vi "Tester.vi"(8 "error in (no error)":errorcluster, 11 "Selector in":refnum<class "Selector.lvclass">) -> (0 "error out":errorcluster, 3 "Selector out":refnum<class "Selector.lvclass">)   [LabVIEW 2019, in "Selector.lvclass"]
uses:
  Selector.lvclass
  Parse/ParseVectorFile/Typedefs/PrivateEvents--ParseVectorFile.NewFile.ctl
  <userlib>/Levylab/Relay Box/Typedefs/Resistor--enum.ctl
  Settings/ObjectSettings/ObjectSettings.lvclass/ObjectSettings.ctl
  Selector.lvclass/Selector.ctl
  <vilib>/Utility/miscctls.llb/LVPositionTypeDef.ctl
  Parse/ParseVectorFile/ParseVectorFile.lvclass
  C:/Program Files/National Instruments/LabVIEW 2019/vi.lib/JKI/JKI SMO/SMO/SMO.lvclass
  Settings/Setting Database/Setting Database.lvclass
  Subpanel/Manager/Subpanel.Edit.lvclass
  C:/Users/Albro/Documents/GitHub/AFM-Lithography/lvsrc/Classes/Subpanel/Subpanel.lvclass
  Tool/Tool Data/Tool Data/Tool Data.lvclass
  Render/BigMAQ/BigMAQ.lvclass
  Parse/ParsePaths/Path.lvclass
  Parse/Rectangle/Rectangle.lvclass
  Parse/Image/SVGImage.lvclass
  Parse/Dot/Dot.lvclass
  Settings/Setting Database/Typedefs/PublicEvents--Setting Database.RectanglesUpdated.ctl
  Settings/Rectangle Settings/Rectangle Settings.lvclass
  C:/Users/Albro/Documents/GitHub/AFM-Lithography/lvsrc/Classes/Settings/ObjectSettings/ObjectSettings.lvclass
  Settings/Setting Database/Typedefs/PublicEvents--Setting Database.PathsUpdated.ctl
  Settings/Path Settings/Path Settings.lvclass
  Settings/Setting Database/Typedefs/PublicEvents--Setting Database.FunnelsUpdated.ctl
  Settings/Funnel Settings/Funnel Settings.lvclass
  Settings/Setting Database/Typedefs/PublicEvents--Setting Database.DotsUpdated.ctl
  Settings/Dot Settings/Dot Settings.lvclass
  Tool/Tool Data/Tool Data/Typedefs/PrivateEvents--Tool Data.Update Objects.ctl
  Settings/Setting Database/Typedefs/PrivateEvents--Setting Database.Refresh.ctl
  Settings/Setting Database/Typedefs/PrivateEvents--Setting Database.Add To Group.ctl
  Settings/Setting Database/Typedefs/PrivateEvents--Setting Database.Create New Group.ctl
  Tool/Tool Path/Tool Path.lvclass
  Tool/Tool Funnel/Tool Funnel.lvclass
  Tool/Tool Rectangle/Tool Rectangle.lvclass
  Tool/Tool Dot/Tool Dots.lvclass
  <vilib>/JKI/JKI SMO/SMO/SMO.lvclass
  Settings/ObjectSettings/ObjectSettings.lvclass
  Subpanel/Subpanel.lvclass
  <userlib>/Levylab/Relay Box/Relay-Box.lvclass
  Identity/Identifier.lvclass
panel:
  in  "Collapse":bool
  out "Render":T1(plugin-control)
  in  "IBW":T2=path "C:/Users/Albro/Documents/GitHub/AFM-Lithography/test files/SA01234A0000.ibw"
  out "Lithography Data":T4(array[cluster])
  out "XY Graph":cluster{"X":dbl, "Y":dbl}[](graph)
  out "Array 2":i32[](array[numeric])
  out "Array":string[](array[string])
  out "Dots":string[](array[string])
  out "Funnels":string[](array[string])
  out "Paths":string[](array[string])
  out "Rectangles":string[](array[string])
  in  "NewFile":T2=path "C:/Users/Albro/Documents/GitHub/AFM-Lithography/test files/test.svg"
  out "Unchanged?":bool
  out "Events":string[](array[string])
  in  "Multicolumn Listbox":i32(listbox)
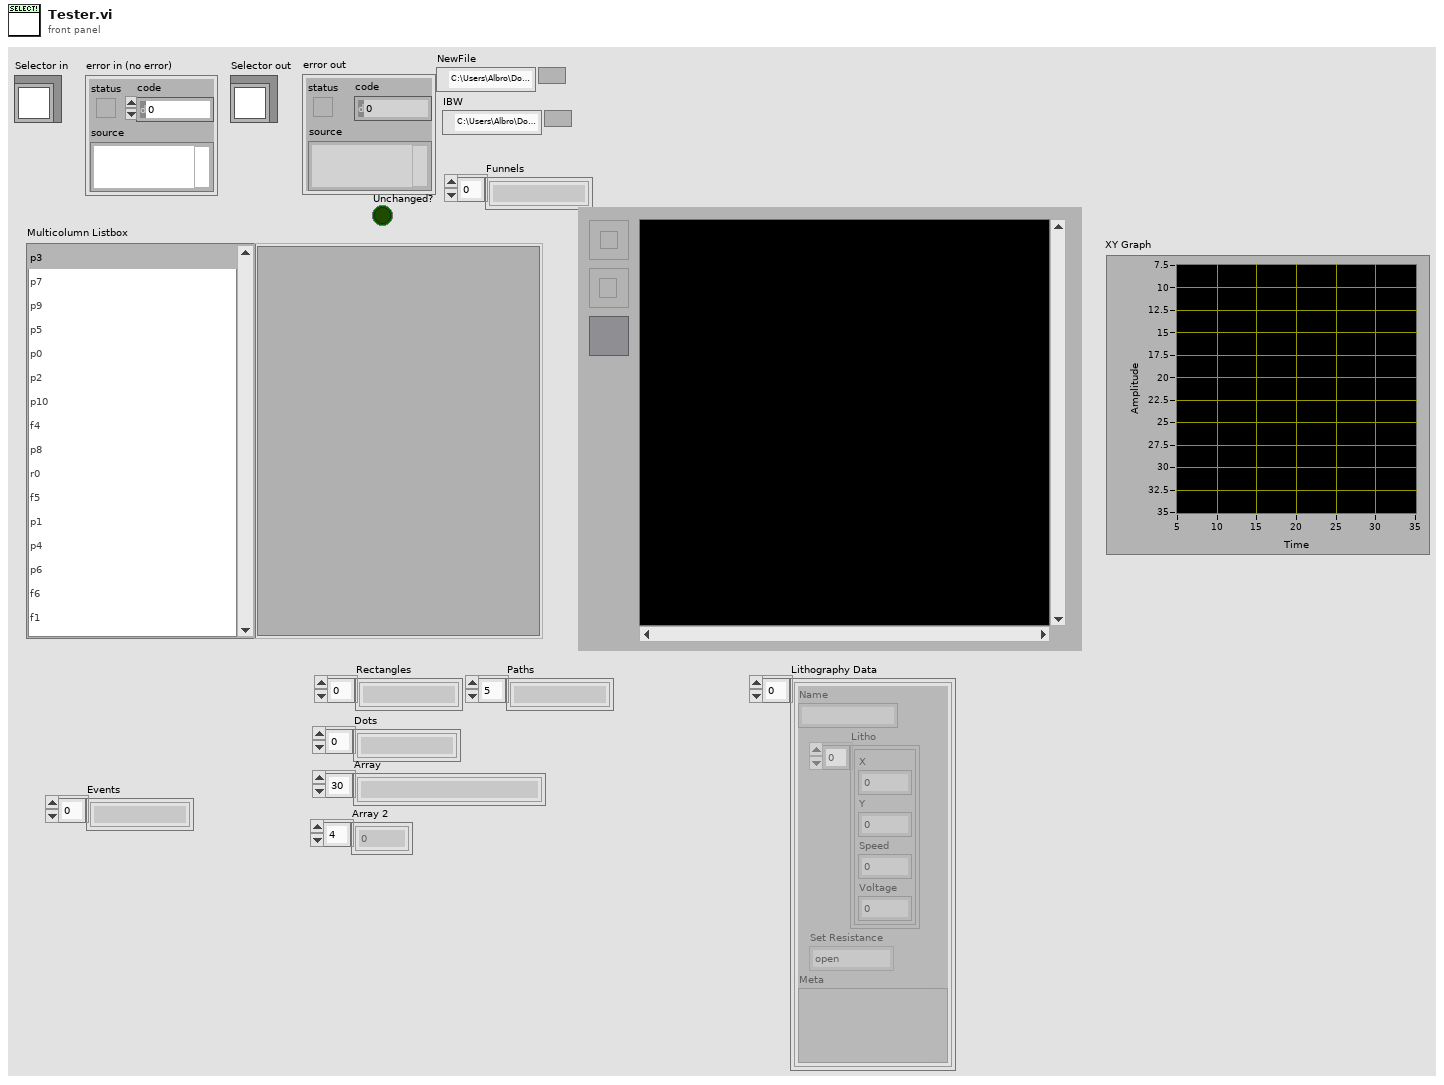
[diagram p1: front panel]
types:
  T1 = typedef "IMAQ Image.ctl" = refnum<image>
  T2 = typedef "ParseVectorFile.lvclass/PrivateEvents--ParseVectorFile.NewFile.ctl" = path
  T3 = typedef "Relay-Box.lvclass/Resistor--enum.ctl" = enum16{"open", "discharge tip", "0 ohms", "100k ohm", "10M ohm", "1G ohm"}
  T4 = cluster{"Name":string, "Litho":cluster{"X":dbl, "Y":dbl, "Speed":dbl, "Voltage":dbl}[], "Set Resistance":T3, "Meta":variant}[]
  T5 = typedef "LVPositionTypeDef.ctl" = cluster{"Left":i32, "Top":i32}
  T6 = cluster{"Point":T5, "Button":u16, "PlatMods":cluster{"Shift":bool, "Ctrl":bool, "Alt":bool, "Cmd":bool, "Opt":bool}}
  T7 = enum32{"Invalid", "Standard", "Closed", "Hidden", "Minimized", "Maximized"}
  T8 = enum32{"invalid app kind", "Development System", "Run Time System", "Student Edition", "Embedded LabVIEW", "Evaluation", "Custom"}
  T9 = cluster{"Name":string, "Group":string, "Enabled":bool}
  T10 = typedef "Tool Data.lvclass/PrivateEvents--Tool Data.Update Objects.ctl" = cluster{"Settings":cluster{"Paths":T11, "Rectangles":T12, "Funnels":T13, "Dots":T14}, "Data":cluster{"Paths":refnum<class "Path.lvclass">[], "Rectangles":refnum<class "Rectangle.lvclass">[], "SVGImage":refnum<class "SVGImage.lvclass">, "Dots":refnum<class "Dot.lvclass">[], "Funnels":refnum<class "Path.lvclass">[]}}
  T11 = typedef "Setting Database.lvclass/PublicEvents--Setting Database.PathsUpdated.ctl" = refnum<class "Path Settings.lvclass">[]
  T12 = typedef "Setting Database.lvclass/PublicEvents--Setting Database.RectanglesUpdated.ctl" = refnum<class "Rectangle Settings.lvclass">[]
  T13 = typedef "Setting Database.lvclass/PublicEvents--Setting Database.FunnelsUpdated.ctl" = refnum<class "Funnel Settings.lvclass">[]
  T14 = typedef "Setting Database.lvclass/PublicEvents--Setting Database.DotsUpdated.ctl" = refnum<class "Dot Settings.lvclass">[]
  T15 = typedef "Setting Database.lvclass/PrivateEvents--Setting Database.Refresh.ctl" = cluster{"Paths":string[], "Rectangles":string[], "Funnels":string[], "Dots":string[]}
  T16 = typedef "Setting Database.lvclass/PrivateEvents--Setting Database.Add To Group.ctl" = cluster{"Name":string, "Group":string}
  T17 = typedef "Setting Database.lvclass/PrivateEvents--Setting Database.Create New Group.ctl" = cluster{"Name":string, "Group":string}
  T18 = cluster{"Paths":refnum<class "Tool Path.lvclass">[], "Funnels":refnum<class "Tool Funnel.lvclass">[], "Rectangles":refnum<class "Tool Rectangle.lvclass">[], "Dots":refnum<class "Tool Dots.lvclass">[]}
  T19 = cluster{"Core":cluster{"Current VI Reference":refnum<vi>, "Close Panel on Exit?":bool}, "menu path":string, "Item Names":string[][], "Settings":refnum<class "Setting Database.lvclass">, "Parser":refnum<class "ParseVectorFile.lvclass">, "Parsed Data":cluster{"Paths":refnum<class "Path.lvclass">[], "Rectangles":refnum<class "Rectangle.lvclass">[], "SVGImage":refnum<class "SVGImage.lvclass">, "Dots":refnum<class "Dot.lvclass">[], "Funnels":refnum<class "Path.lvclass">[]}, "GUIDs":cluster{"Dots":string[], "Funnels":string[], "Rects":string[], "Paths":string[]}, "Subpanel.Edit":refnum<class "Subpanel.Edit.lvclass">, "Tooler":refnum<class "Tool Data.lvclass">, "Obj Settings":cluster{"Rectangles":T12, "Paths":T11, "Funnels":T13, "Dots":T14}, "Lithography Data":cluster{"Name":string, "Litho":cluster{"X":dbl, "Y":dbl, "Speed":dbl, "Voltage":dbl}[], "Set Resistance":T3, "Meta":variant}[], "BigMAQ":refnum<class "BigMAQ.lvclass">, "Changed Objects":cluster{"Path Changes":cluster{bool, "index of element":i32}[], "Funnel Changes":cluster{bool, "index of element":i32}[], "Rectangle Changes":cluster{bool, "index of element":i32}[], "Dot Changes":cluster{bool, "index of element":i32}[]}}
  T20 = typedef "LVPoint32TypeDef.ctl" = cluster{"Horizontal":i32, "Vertical":i32}
  T21 = cluster{"Shift":bool, "Ctrl":bool, "Alt":bool, "Cmd":bool, "Opt":bool}
  T22 = cluster{"Path Changes":cluster{bool, "index of element":i32}[], "Funnel Changes":cluster{bool, "index of element":i32}[], "Rectangle Changes":cluster{bool, "index of element":i32}[], "Dot Changes":cluster{bool, "index of element":i32}[]}
  T23 = cluster{"Rectangles":T12, "Paths":T11, "Funnels":T13, "Dots":T14}
  T24 = cluster{"Dots":string[], "Funnels":string[], "Rects":string[], "Paths":string[]}
  T25 = cluster{"Paths":refnum<class "Path.lvclass">[], "Rectangles":refnum<class "Rectangle.lvclass">[], "SVGImage":refnum<class "SVGImage.lvclass">, "Dots":refnum<class "Dot.lvclass">[], "Funnels":refnum<class "Path.lvclass">[]}
  T26 = cluster{"Current VI Reference":refnum<vi>, "Close Panel on Exit?":bool}
  T27 = typedef "Tool Data.lvclass/PublicEvents--Cluster.ctl" = cluster{"Objects Updated":refnum<user-event>}
  T28 = typedef "ParseVectorFile.lvclass/PublicEvents--Cluster.ctl" = cluster{"ParsedData":refnum<user-event>}
  T29 = typedef "Setting Database.lvclass/PublicEvents--Cluster.ctl" = cluster{"NewActivePath":refnum<user-event>, "PathsUpdated":refnum<user-event>, "RectanglesUpdated":refnum<user-event>, "NewActiveRectangle":refnum<user-event>, "NewActiveFunnel":refnum<user-event>, "FunnelsUpdated":refnum<user-event>, "NewActiveDot":refnum<user-event>, "DotsUpdated":refnum<user-event>}
  T30 = typedef "Selector.lvclass/Item.ctl" = cluster{"Name":string, "Group":string, "Enabled":bool}
  T31 = cluster{"X":dbl, "Y":dbl, "Speed":dbl, "Voltage":dbl}[]
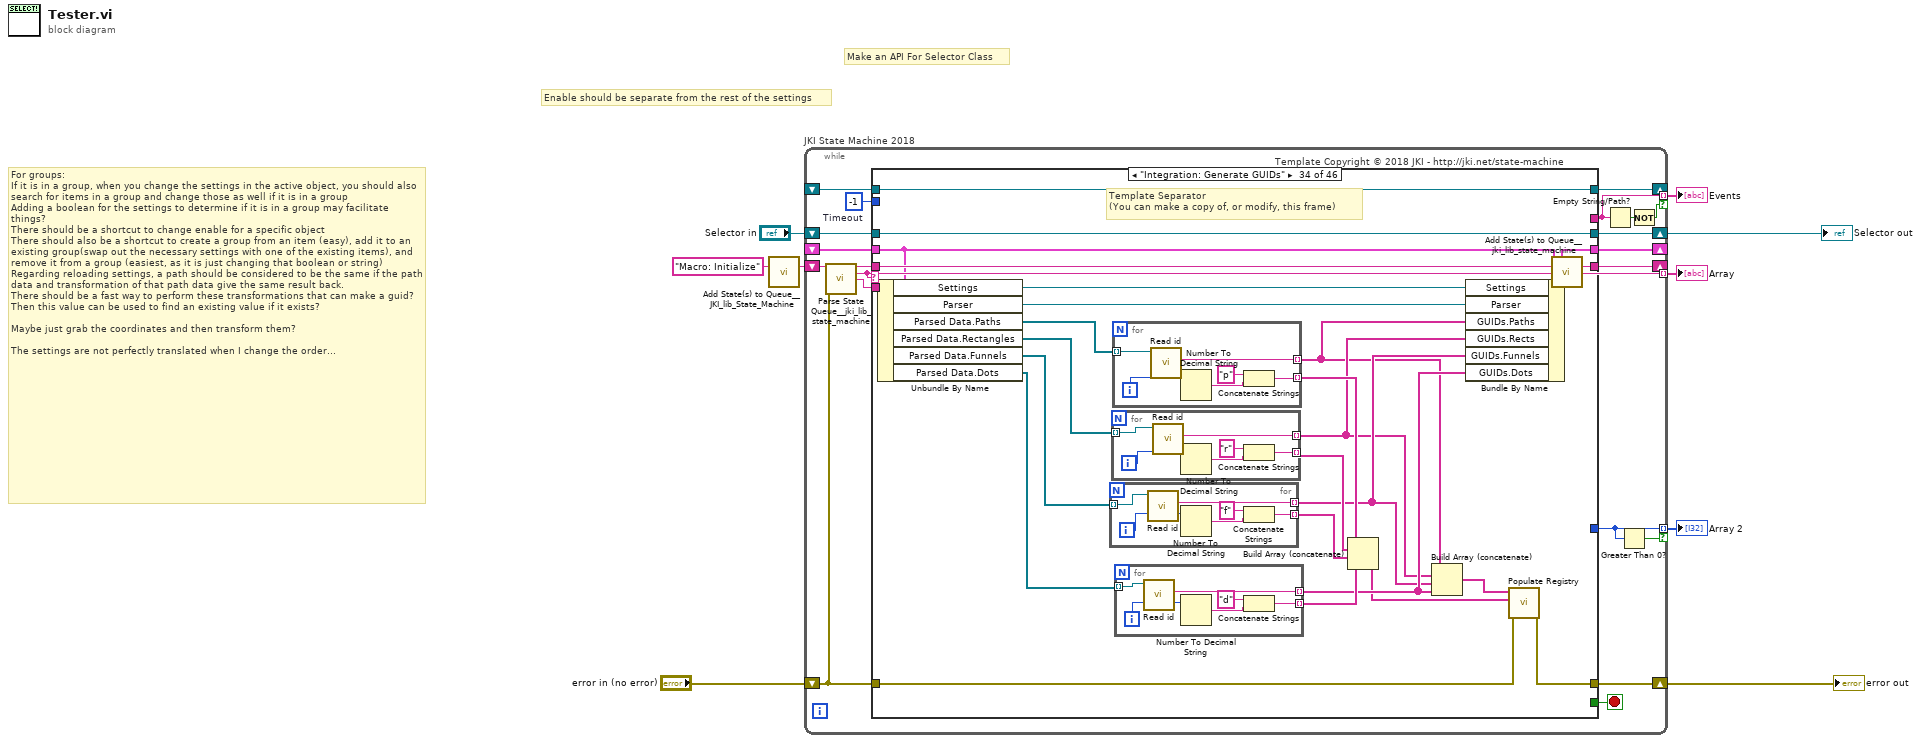
[diagram p0: block diagram]
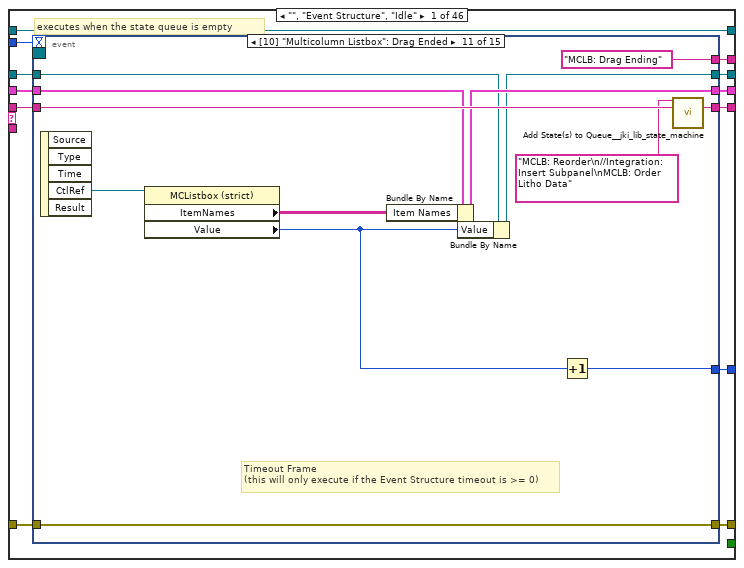
[diagram p2: hidden frame]
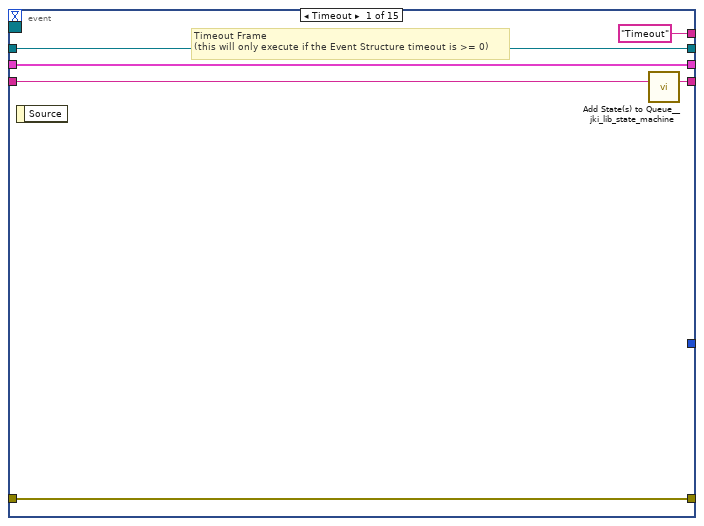
[diagram p3: hidden frame]
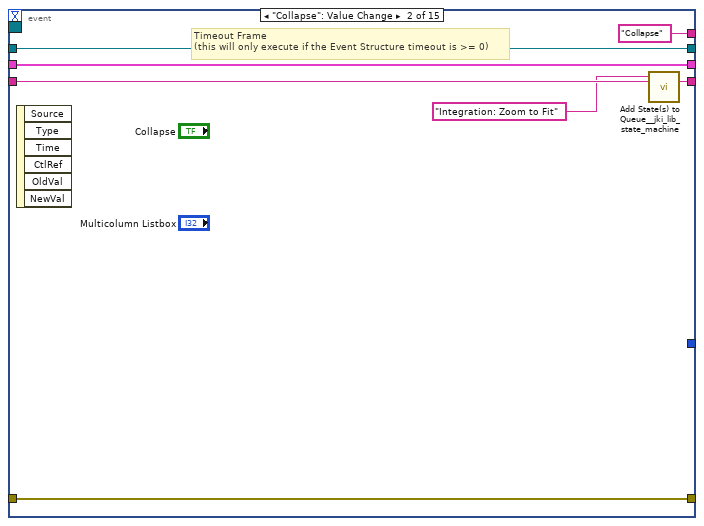
[diagram p4: hidden frame]
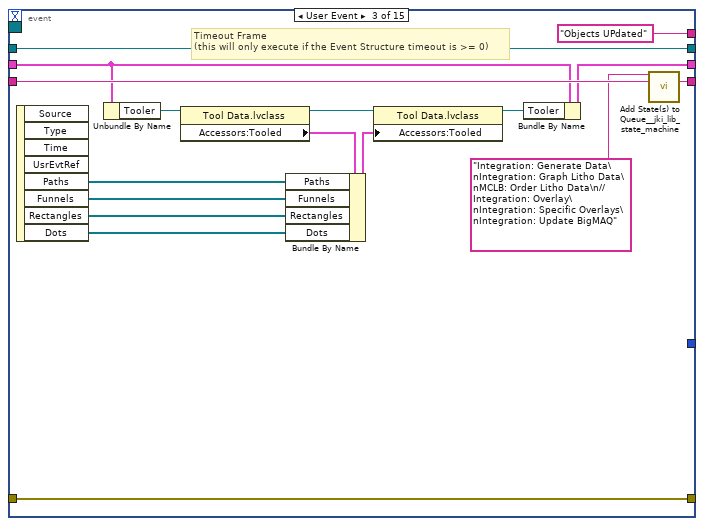
[diagram p5: hidden frame]
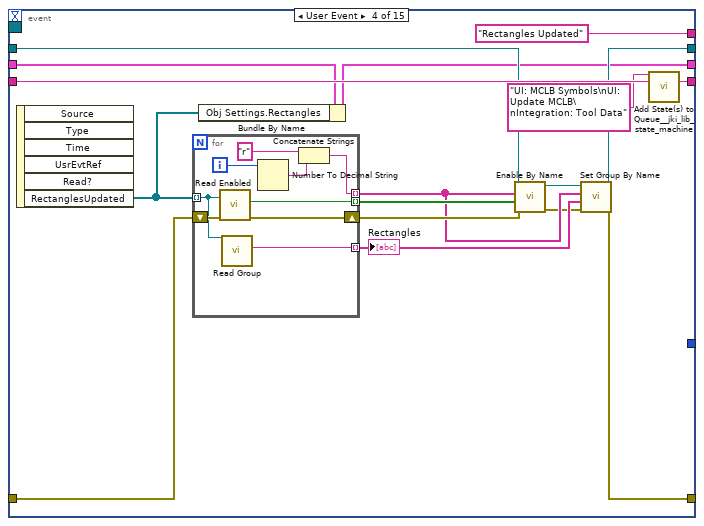
[diagram p6: hidden frame]
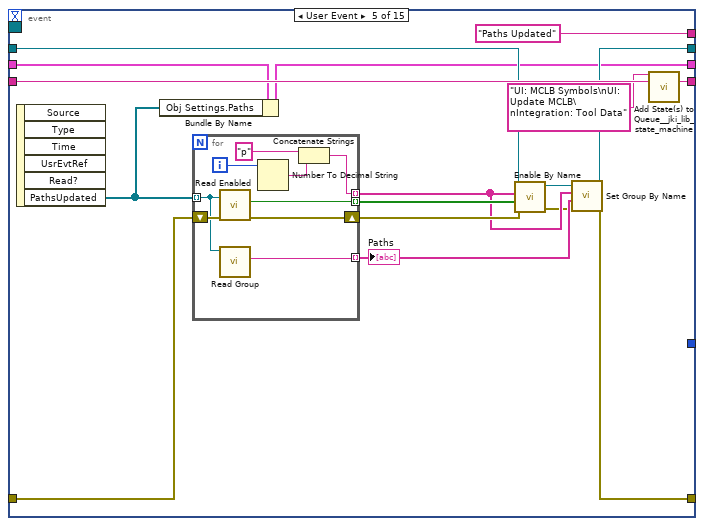
[diagram p7: hidden frame]
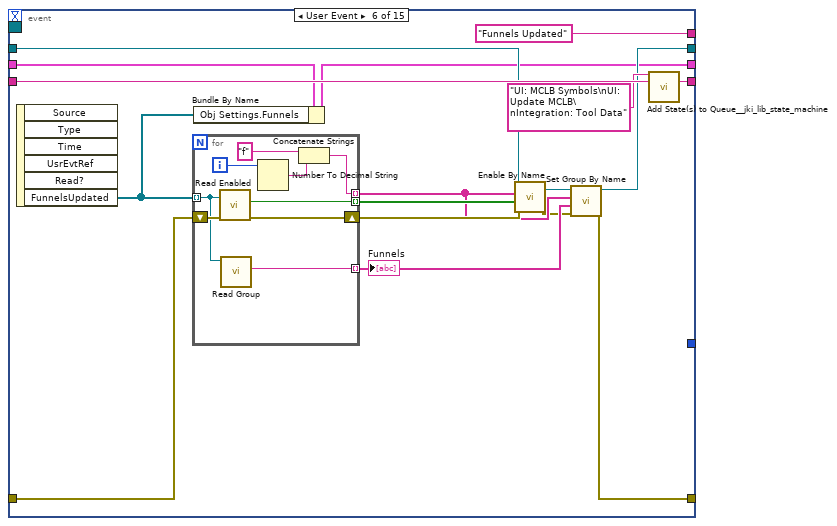
[diagram p8: hidden frame]
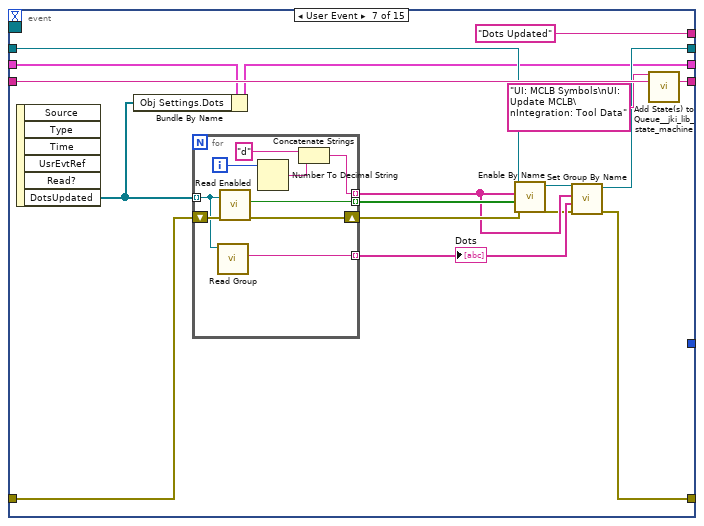
[diagram p9: hidden frame]
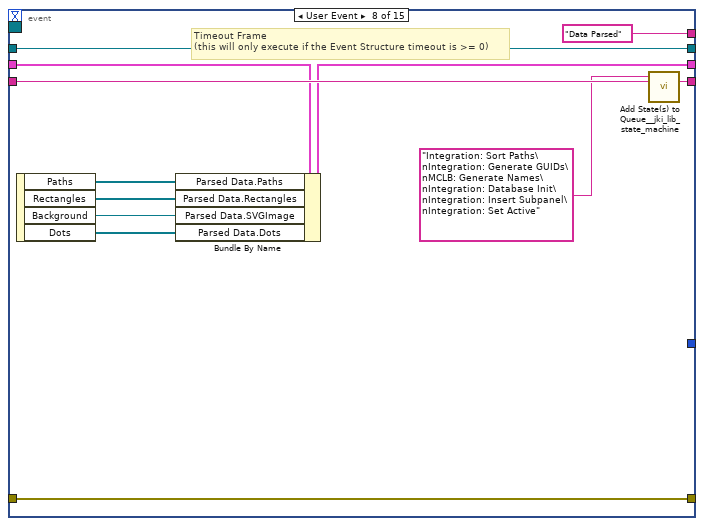
[diagram p10: hidden frame]
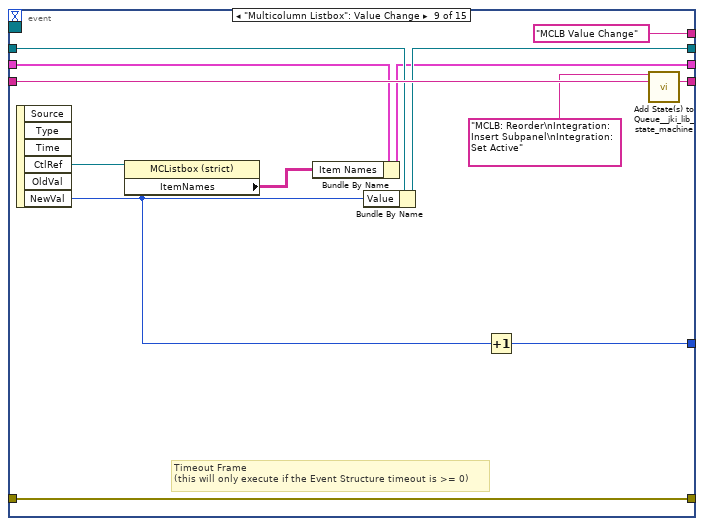
[diagram p11: hidden frame]
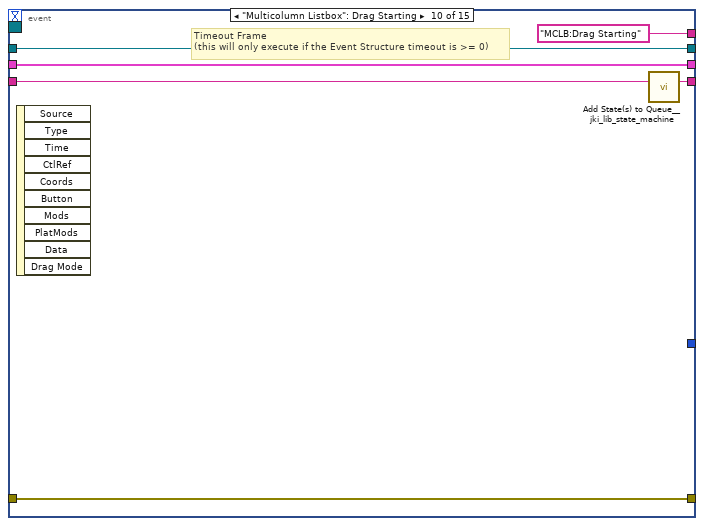
[diagram p12: hidden frame]
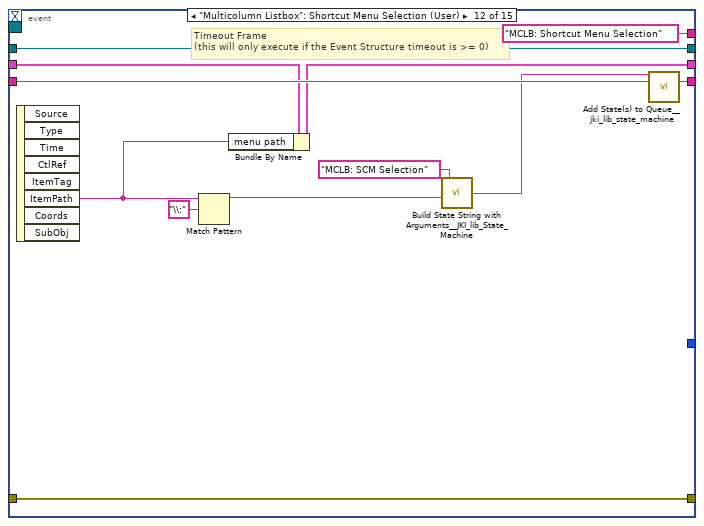
[diagram p13: hidden frame]
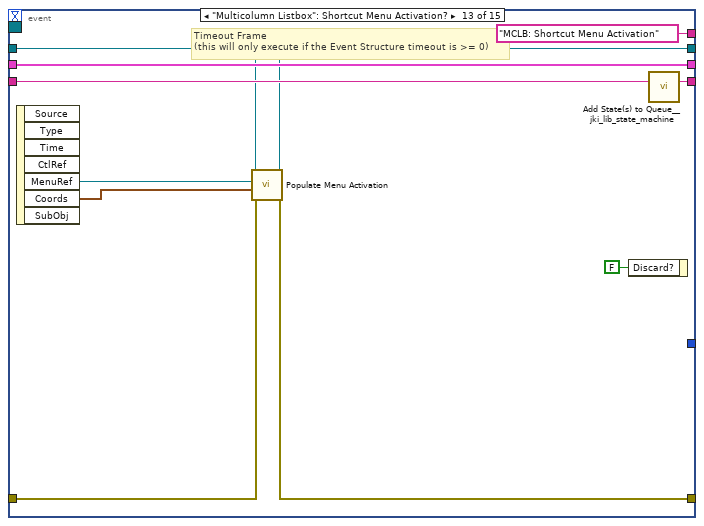
[diagram p14: hidden frame]
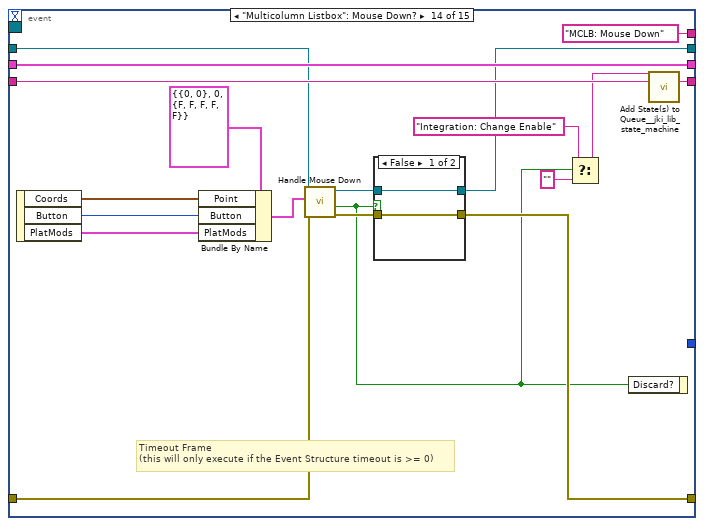
[diagram p15: hidden frame]
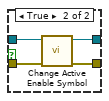
[diagram p16: hidden frame]
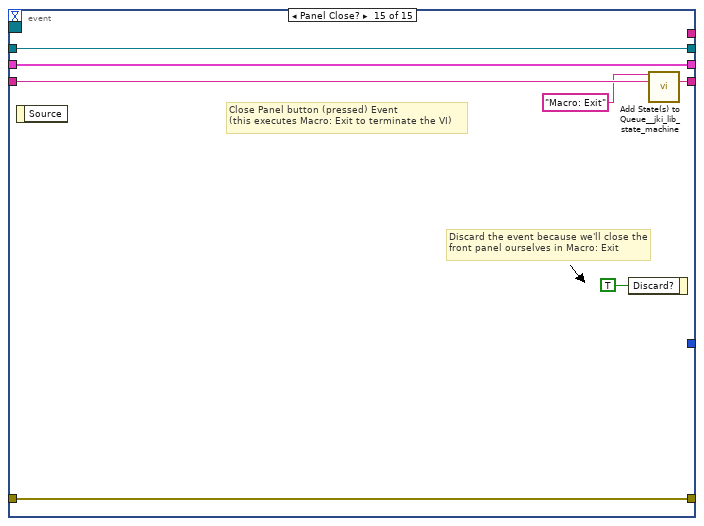
[diagram p17: hidden frame]
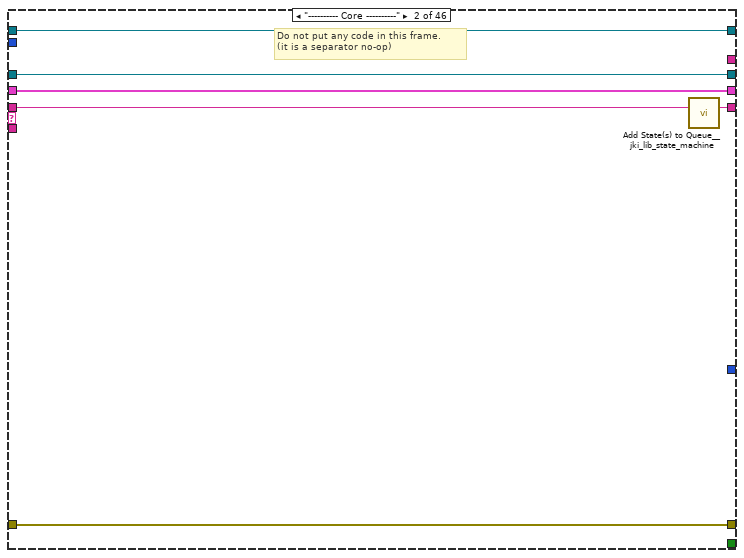
[diagram p18: hidden frame]
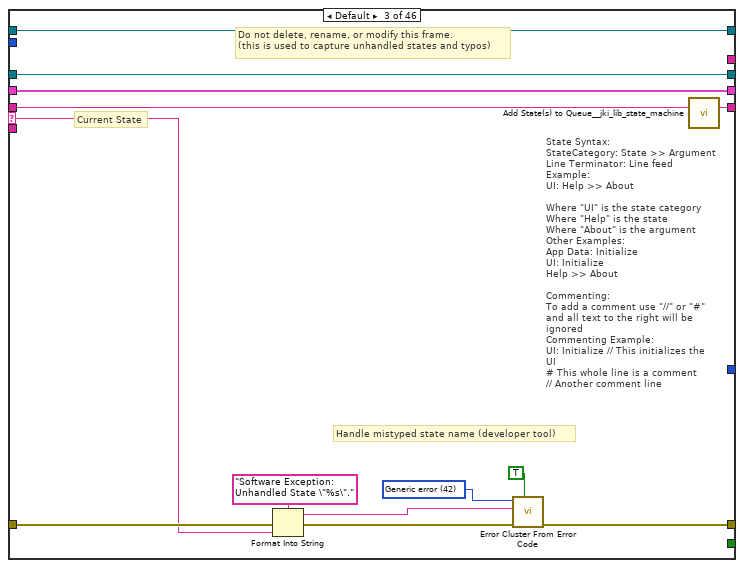
[diagram p19: hidden frame]
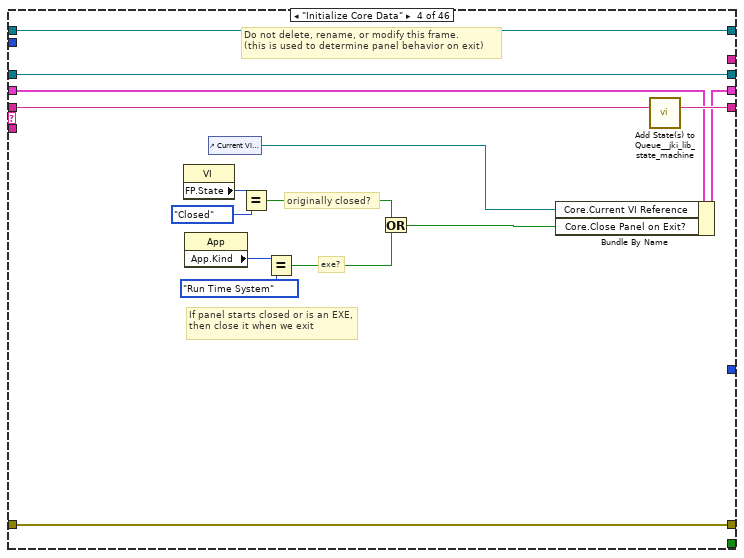
[diagram p20: hidden frame]
diagram:
  # "Make an API For Selector Class"
  # "For groups:\nIf it is in a group, when you change the settings in the active object, you should also search for items in a group and change those as well if it is in a group \nAdding a boolean for the settings to determine if it is in a group may facilitate things?\nThere should be a shortcut to change enable for a specific object\nThere should also be a shortcut to create a group from an item (easy), add it to an existing group(swap out the necessary settings with one of the existing items), and remove it from a group (easiest, as it is just changing that boolean or string)\nRegarding reloading settings, a path should be considered to be the same if the path data and transformation of that path data give the same result back.\nThere should be a fast way to perform these transformations that can make a guid? Then this value can be used to find an existing value if it exists?\n\nMaybe just grab the coordinates and then transform them?\n\nThe settings are not perfectly translated when I change the order..."
  # "Enable should be separate from the rest of the settings"
  n1 = call <vilib>:"Add State(s) to Queue__JKI_lib_State_Machine.vi"("State(s) in (\"\")"="Macro: Initialize") -> ("States Out"=w9:string)  [unwired: 14 in]
  n2 = while "JKI State Machine 2018" {
    shift-right: [w23] -> _
    shift-left: _ -> [w22]
    shift-right: [w26] -> w4
    shift-left: "error in (no error)" -> [w20]
    shift-right: [w25] -> _
    shift-left: w9 -> [w27]
    shift-right: [w18] -> w6
    shift-left: "Selector in" -> [w19]
    tunnel: [w17] -> w3 mode=indexing if=w12
    shift-right: [w15] -> _
    shift-left: _ -> [w14]
    tunnel: [w13] -> w2 mode=indexing
    tunnel: [w11] -> w1 mode=indexing if=w10
    stop <- w24 stop-if-true
    w21 = -1  # Timeout
    # "Template Copyright © 2018 JKI - http://jki.net/state-machine"
    n3 = call <vilib>:"Parse State Queue__jki_lib_state_machine.vi"("State Queue"=w27, "Error In (no error)"=w20) -> ("Remaining States"=w29:string, "Current State"=w13:string, "Arguments"=w28:string)  [unwired: 11 in]
    n4 = case shown="\"Integration: Generate GUIDs\"" w13 {
      selector: w13 -> [_ _ w283 _ _ _ _ _ _ _ _ _ _ _ _ _ _ _ _ _ _ _ _ _ _ _ _ _ _ _ _ _ _ _ _ _ _ _ _ _ _ _ _ _ _ _]
      tunnel: w29 -> [w41 w280 w287 w308 w316 w323 w329 w342 w367 w377 w383 w400 w407 w413 w423 w441 w449 w462 w535 w541 w548 w560 w571 w590 w613 w628 w641 w658 w668 w688 w712 w731 w769 w793 w832 w852 w864 w884 w906 w937 w943 w958 w984 w1006 w1023 w1036]
      tunnel: w28 -> [_ _ _ _ _ _ _ _ _ _ _ _ _ _ _ _ w444 w456 _ _ _ _ _ _ _ _ _ _ _ _ _ _ _ _ _ _ _ _ _ _ _ _ _ _ _ w1034]
      tunnel: w22 -> [w39 w277 w285 w301 w313 w321 w326 w339 _ w373 w380 w395 w405 w410 w421 w433 w447 w458 w533 w538 w545 w557 w566 w585 w608 w623 w636 w653 w663 w683 w707 w727 w765 w788 w828 w847 w859 w878 w901 w932 w940 w946 w980 w1003 w1017 w1024]
      tunnel: [w38 w278 w289 w305 errorcluster {"status"=FALSE, "code"=0, "source"=""} ("error out") w320 w327 w340 w362 w374 w381 w389 w401 w411 w415 w425 w445 w459 w528 w539 w546 w558 w561 w581 w602 w616 w630 w642 w666 w678 w696 w718 w754 w777 w819 w836 w854 w874 w892 w923 w941 w949 w982 w1004 w1019 w1031] -> w26
      tunnel: w20 -> [w37 w278 w288 w305 w312 w320 w327 w340 w362 w368 w381 w390 w402 w411 w414 w432 w446 w460 w529 w539 w546 w558 w561 w581 w601 w615 w629 w647 w666 w677 w695 w714 w755 w776 w818 w835 w853 w873 w888 w907 w941 w951 w982 w1004 w1018 w1030]
      tunnel: [w40 w279 w286 w307 w315 w322 w328 w341 w366 w376 w382 w399 w406 w412 w422 w440 w448 w461 w534 w540 w547 w559 w570 w589 w612 w627 w640 w657 w667 w687 w711 w730 w768 w792 w831 w851 w863 w883 w905 w936 w942 w957 w983 w1005 w1022 w1035] -> w25
      tunnel: [_ _ _ _ _ TRUE _ _ _ _ _ _ _ _ _ _ _ _ _ _ _ _ _ _ _ _ _ _ _ _ _ _ _ _ _ _ _ _ _ _ _ _ _ _ _ _] -> w24
      tunnel: [w36 w277 w285 w306 w313 w321 w326 w339 w365 w373 w380 w395 w405 w410 w421 w434 w447 w458 w533 w538 w545 w557 w567 w586 w609 w624 w637 w654 w663 w684 w708 w728 w766 w789 w829 w848 w860 w881 w902 w933 w940 w947 w980 w1003 w1017 w1026] -> w23
      tunnel: w21 -> [w35 _ _ _ _ _ _ _ _ _ _ _ _ _ _ _ _ _ _ _ _ _ _ _ _ _ _ _ _ _ _ _ _ _ _ _ _ _ _ _ _ _ _ _ _ _]
      tunnel: w19 -> [w34 w276 w282 w295 w310 w318 w325 w330 w361 w372 w379 w398 w404 w409 w419 w439 w443 w455 w530 w537 w543 w550 w569 w588 w611 w626 w639 w656 w665 w686 w710 w719 w763 w791 w824 w850 w862 w866 w904 w935 w939 w955 w968 w996 w1020 w1025]
      tunnel: [w33 w276 w282 w295 w310 w318 w325 w331 w361 w372 w379 w398 w404 w409 w419 w435 w443 w455 w532 w537 w543 w550 w569 w588 w611 w626 w639 w656 w665 w686 w710 w719 w763 w791 w824 w850 w862 w867 w904 w935 w939 w948 w969 w997 w1021 w1033] -> w18
      tunnel: [w32 _ _ _ _ _ _ _ _ _ _ _ _ _ _ _ _ _ _ _ _ _ _ _ _ _ _ _ _ _ _ _ _ _ _ _ _ _ _ _ _ _ _ _ _ _] -> w17
      tunnel: [w31 w275 w281 w294 w309 w317 w324 w338 w363 w371 w378 w397 w403 w408 w420 w438 w442 w454 w531 w536 w542 w549 w568 w587 w610 w625 w638 w655 w664 w685 w709 w729 w767 w790 w830 w849 w861 w882 w903 w934 w938 w956 w981 w994 w1012 w1029] -> w15
      tunnel: w14 -> [w31 w275 w281 w294 w309 w317 w324 w338 w363 w371 w378 _ w403 w408 w420 w438 w442 w454 w531 w536 w542 w549 w568 w587 w610 w625 w638 w655 w664 w685 w709 w729 w767 w790 w830 w849 w861 w882 w903 w934 w938 w956 w981 w994 w1012 w1029]
      tunnel: [w30 _ _ _ _ _ _ _ _ _ _ _ _ _ _ _ _ _ _ _ _ _ _ _ _ _ _ _ _ _ _ _ _ _ _ _ _ _ _ _ _ _ _ _ _ _] -> w11
      frame "", "Event Structure", "Idle" {
        # "executes when the state queue is empty"
        n5 = event shown="[10] \"Multicolumn Listbox\": Drag Ended" {
          selector: w31 -> [_ _ _ _ _ _ _ _ _ _ _ _ _ _ _]
          dyn-events: _ -> [_ _ _ _ _ _ _ _ _ _ _ _ _ _ _]
          timeout: w35 -> [_ _ _ _ _ _ _ _ _ _ _ _ _ _ _]
          tunnel: w41 -> [w47 w54 w71 w88 w114 w140 w166 w187 w200 w206 w219 w231 w242 w261 w274]
          tunnel: [w46 w53 w70 w87 w113 w139 w165 w186 w199 w205 w218 w230 w241 w260 w273] -> w40
          tunnel: w39 -> [w44 w51 w65 w73 w99 w125 w151 w177 w189 w203 w211 w224 w240 w259 w271]
          tunnel: [w45 w52 w69 w76 w103 w127 w153 w185 w198 w204 w217 w229 w235 w251 w272] -> w38
          tunnel: w37 -> [w45 w52 w69 w82 w108 w134 w160 w185 w198 w204 w217 w229 w234 w257 w272]
          tunnel: [w44 w51 w66 w74 w100 w126 w152 w182 w190 w203 w212 w225 w240 w259 w271] -> w36
          tunnel: w34 -> [w43 w50 w68 w75 w107 w133 w159 w184 w195 w202 w209 w228 w232 w258 w268]
          tunnel: [w43 w50 w68 w80 w101 w131 w157 w184 w196 w202 w210 w228 w239 w249 w268] -> w33
          tunnel: ["Timeout" "Collapse" "Objects UPdated" "Rectangles Updated" "Paths Updated" "Funnels Updated" "Dots Updated" "Data Parsed" "MCLB Value Change" "MCLB:Drag Starting" "MCLB: Drag Ending" "MCLB: Shortcut Menu Selection" "MCLB: Shortcut Menu Activation" "MCLB: Mouse Down" _] -> w32
          tunnel: [_ _ _ _ _ _ _ _ w192 _ w207 _ _ _ _] -> w30
          event Timeout {
            # "Timeout Frame\n(this will only execute if the Event Structure timeout is >= 0)"
            n6 = event-data() -> ()  [unwired: 1 in, 1 out]
            n7 = call <vilib>:"Add State(s) to Queue__jki_lib_state_machine.vi"("State(s) in (\"\")"=w47) -> ("States Out"=w46:string)  [unwired: 14 in]
          }
          event "Collapse": Value Change {
            # "Timeout Frame\n(this will only execute if the Event Structure timeout is >= 0)"
            n8 = event-data() -> ()  [unwired: 1 in, 6 out]
            n9 = call <vilib>:"Add State(s) to Queue__jki_lib_state_machine.vi"("State(s) in Front (\"\")"="Integration: Zoom to Fit", "State(s) in (\"\")"=w54) -> ("States Out"=w53:string)  [unwired: 13 in]
          }
          event User Event {
            # "Timeout Frame\n(this will only execute if the Event Structure timeout is >= 0)"
            n10 = event-data() -> ("Paths"=w61:refnum<class "Tool Path.lvclass">[], "Funnels"=w60:refnum<class "Tool Funnel.lvclass">[], "Rectangles"=w59:refnum<class "Tool Rectangle.lvclass">[], "Dots"=w58:refnum<class "Tool Dots.lvclass">[])  [unwired: 1 in, 4 out]
            n11 = Unbundle By Name(w65) -> ("Tooler"=w56:refnum<class "Tool Data.lvclass">)
            n12 = property class="Tool Data.lvclass"(reference=w56) -> (reference out=w64:refnum<class "Tool Data.lvclass">, "Accessors:Tooled"=w62:T18)  [unwired: 1 in, 1 out]
            n13 = Bundle By Name(cluster=w62, "Paths"=w61, "Funnels"=w60, "Rectangles"=w59, "Dots"=w58) -> (w55:T18)
            n14 = property class="Tool Data.lvclass"(reference=w64, "Accessors:Tooled"=w55) -> (reference out=w63:refnum<class "Tool Data.lvclass">)  [unwired: 1 in, 1 out]
            n15 = Bundle By Name(cluster=w65, "Tooler"=w63) -> (w66:T19)
            n16 = call <vilib>:"Add State(s) to Queue__jki_lib_state_machine.vi"("State(s) in Front (\"\")"="Integration: Generate Data\nIntegration: Graph Litho Data\nMCLB: Order Litho Data\n//Integration: Overlay\nIntegration: Specific Overlays\nIntegration: Update BigMAQ" ("State(s) in Front (\"\")"), "State(s) in (\"\")"=w71) -> ("States Out"=w70:string)  [unwired: 13 in]
          }
          event User Event {
            n17 = event-data() -> ("RectanglesUpdated"=w72:T12)  [unwired: 1 in, 5 out]
            n18 = for {
              tunnel: w72 -> [w90] mode=indexing
              tunnel: [w97] -> w84 mode=indexing
              tunnel: [w93] -> w79 mode=indexing
              shift-right: [w92] -> w83
              shift-left: w82 -> [w91]
              tunnel: [w89] -> w78 mode=indexing
              i -> [w95]
              n19 = call "Read Enabled.vi"("error in (no error)"=w91, "ObjectSettings in"=w90) -> ("error out"=w92:errorcluster, "Enabled"=w97:bool)  [unwired: 7 in, 1 out]
              n20 = call-dynamic "Read Group.vi"("ObjectSettings in"=w90) -> ("Group"=w89:string)  [unwired: 8 in, 2 out]
              n21 = Number To Decimal String(number=w95) -> (decimal integer string=w94:string)  [unwired: 1 in]
              n22 = Concatenate Strings("r" ("string"), w94) -> (w93:string)
            }
            "Rectangles" <- w78
            n23 = Bundle By Name(cluster=w73, "Obj Settings.Rectangles"=w72) -> (w74:T19)
            n24 = call-dynamic "Enable By Name.vi"("error in (no error)"=w83, "Enable Items"=w84, "Names"=w79, "Selector in"=w75) -> ("error out"=w77:errorcluster, "Selector out"=w81:refnum<class "Selector.lvclass">)  [unwired: 6 in]
            n25 = call "Set Group By Name.vi"("error in (no error)"=w77, "Groups"=w78, "Names"=w79, "Selector in"=w81) -> ("error out"=w76:errorcluster, "Selector out"=w80:refnum<class "Selector.lvclass">)  [unwired: 6 in]
            n26 = call <vilib>:"Add State(s) to Queue__jki_lib_state_machine.vi"("State(s) in Front (\"\")"="UI: MCLB Symbols\nUI: Update MCLB\nIntegration: Tool Data", "State(s) in (\"\")"=w88) -> ("States Out"=w87:string)  [unwired: 13 in]
          }
          event User Event {
            n27 = event-data() -> ("PathsUpdated"=w98:T11)  [unwired: 1 in, 5 out]
            n28 = Bundle By Name(cluster=w99, "Obj Settings.Paths"=w98) -> (w100:T19)
            n29 = for {
              tunnel: w98 -> [w116] mode=indexing
              tunnel: [w123] -> w110 mode=indexing
              tunnel: [w119] -> w106 mode=indexing
              shift-right: [w118] -> w109
              shift-left: w108 -> [w117]
              tunnel: [w115] -> w105 mode=indexing
              i -> [w121]
              n30 = call "Read Enabled.vi"("error in (no error)"=w117, "ObjectSettings in"=w116) -> ("error out"=w118:errorcluster, "Enabled"=w123:bool)  [unwired: 7 in, 1 out]
              n31 = call-dynamic "Read Group.vi"("ObjectSettings in"=w116) -> ("Group"=w115:string)  [unwired: 8 in, 2 out]
              n32 = Number To Decimal String(number=w121) -> (decimal integer string=w120:string)  [unwired: 1 in]
              n33 = Concatenate Strings("p" ("string"), w120) -> (w119:string)
            }
            "Paths" <- w105
            n34 = call-dynamic "Enable By Name.vi"("error in (no error)"=w109, "Enable Items"=w110, "Names"=w106, "Selector in"=w107) -> ("error out"=w104:errorcluster, "Selector out"=w102:refnum<class "Selector.lvclass">)  [unwired: 6 in]
            n35 = call "Set Group By Name.vi"("error in (no error)"=w104, "Groups"=w105, "Names"=w106, "Selector in"=w102) -> ("error out"=w103:errorcluster, "Selector out"=w101:refnum<class "Selector.lvclass">)  [unwired: 6 in]
            n36 = call <vilib>:"Add State(s) to Queue__jki_lib_state_machine.vi"("State(s) in Front (\"\")"="UI: MCLB Symbols\nUI: Update MCLB\nIntegration: Tool Data", "State(s) in (\"\")"=w114) -> ("States Out"=w113:string)  [unwired: 13 in]
          }
          event User Event {
            n37 = event-data() -> ("FunnelsUpdated"=w124:T13)  [unwired: 1 in, 5 out]
            n38 = for {
              tunnel: w124 -> [w142] mode=indexing
              tunnel: [w149] -> w136 mode=indexing
              tunnel: [w145] -> w130 mode=indexing
              shift-right: [w144] -> w135
              shift-left: w134 -> [w143]
              tunnel: [w141] -> w129 mode=indexing
              i -> [w147]
              n39 = call "Read Enabled.vi"("error in (no error)"=w143, "ObjectSettings in"=w142) -> ("error out"=w144:errorcluster, "Enabled"=w149:bool)  [unwired: 7 in, 1 out]
              n40 = call-dynamic "Read Group.vi"("ObjectSettings in"=w142) -> ("Group"=w141:string)  [unwired: 8 in, 2 out]
              n41 = Number To Decimal String(number=w147) -> (decimal integer string=w146:string)  [unwired: 1 in]
              n42 = Concatenate Strings("f" ("string"), w146) -> (w145:string)
            }
            "Funnels" <- w129
            n43 = Bundle By Name(cluster=w125, "Obj Settings.Funnels"=w124) -> (w126:T19)
            n44 = call-dynamic "Enable By Name.vi"("error in (no error)"=w135, "Enable Items"=w136, "Names"=w130, "Selector in"=w133) -> ("error out"=w128:errorcluster, "Selector out"=w132:refnum<class "Selector.lvclass">)  [unwired: 6 in]
            n45 = call "Set Group By Name.vi"("error in (no error)"=w128, "Groups"=w129, "Names"=w130, "Selector in"=w132) -> ("error out"=w127:errorcluster, "Selector out"=w131:refnum<class "Selector.lvclass">)  [unwired: 6 in]
            n46 = call <vilib>:"Add State(s) to Queue__jki_lib_state_machine.vi"("State(s) in Front (\"\")"="UI: MCLB Symbols\nUI: Update MCLB\nIntegration: Tool Data", "State(s) in (\"\")"=w140) -> ("States Out"=w139:string)  [unwired: 13 in]
          }
          event User Event {
            n47 = event-data() -> ("DotsUpdated"=w150:T14)  [unwired: 1 in, 5 out]
            n48 = Bundle By Name(cluster=w151, "Obj Settings.Dots"=w150) -> (w152:T19)
            n49 = for {
              tunnel: w150 -> [w168] mode=indexing
              tunnel: [w175] -> w162 mode=indexing
              tunnel: [w171] -> w156 mode=indexing
              shift-right: [w170] -> w161
              shift-left: w160 -> [w169]
              tunnel: [w167] -> w155 mode=indexing
              i -> [w173]
              n50 = call-dynamic "Read Group.vi"("ObjectSettings in"=w168) -> ("Group"=w167:string)  [unwired: 8 in, 2 out]
              n51 = call "Read Enabled.vi"("error in (no error)"=w169, "ObjectSettings in"=w168) -> ("error out"=w170:errorcluster, "Enabled"=w175:bool)  [unwired: 7 in, 1 out]
              n52 = Number To Decimal String(number=w173) -> (decimal integer string=w172:string)  [unwired: 1 in]
              n53 = Concatenate Strings("d" ("string"), w172) -> (w171:string)
            }
            "Dots" <- w155
            n54 = call-dynamic "Enable By Name.vi"("error in (no error)"=w161, "Enable Items"=w162, "Names"=w156, "Selector in"=w159) -> ("error out"=w154:errorcluster, "Selector out"=w158:refnum<class "Selector.lvclass">)  [unwired: 6 in]
            n55 = call "Set Group By Name.vi"("error in (no error)"=w154, "Groups"=w155, "Names"=w156, "Selector in"=w158) -> ("error out"=w153:errorcluster, "Selector out"=w157:refnum<class "Selector.lvclass">)  [unwired: 6 in]
            n56 = call <vilib>:"Add State(s) to Queue__jki_lib_state_machine.vi"("State(s) in Front (\"\")"="UI: MCLB Symbols\nUI: Update MCLB\nIntegration: Tool Data", "State(s) in (\"\")"=w166) -> ("States Out"=w165:string)  [unwired: 13 in]
          }
          event User Event {
            # "Timeout Frame\n(this will only execute if the Event Structure timeout is >= 0)"
            n57 = event-data() -> ("Paths"=w181:refnum<class "Path.lvclass">[], "Rectangles"=w180:refnum<class "Rectangle.lvclass">[], "Background"=w179:refnum<class "SVGImage.lvclass">, "Dots"=w178:refnum<class "Dot.lvclass">[])  [unwired: 1 in]
            n58 = Bundle By Name(cluster=w177, "Parsed Data.Paths"=w181, "Parsed Data.Rectangles"=w180, "Parsed Data.SVGImage"=w179, "Parsed Data.Dots"=w178) -> (w182:T19)
            n59 = call <vilib>:"Add State(s) to Queue__jki_lib_state_machine.vi"("State(s) in Front (\"\")"="Integration: Sort Paths\nIntegration: Generate GUIDs\nMCLB: Generate Names\nIntegration: Database Init\nIntegration: Insert Subpanel\nIntegration: Set Active", "State(s) in (\"\")"=w187) -> ("States Out"=w186:string)  [unwired: 13 in]
          }
          event "Multicolumn Listbox": Value Change {
            # "Timeout Frame\n(this will only execute if the Event Structure timeout is >= 0)"
            n60 = event-data() -> ("CtlRef"=w191:refnum<vi>, "NewVal"=w193:i32)  [unwired: 1 in, 4 out]
            n61 = property class="MCListbox (strict)"(reference=w191) -> ("ItemNames"=w188:string[][])  [unwired: 1 in, 2 out]
            n62 = Bundle By Name(cluster=w189, "Item Names"=w188) -> (w190:T19)
            n63 = Bundle By Name(cluster=w195, "Value"=w193) -> (w196:refnum<class "Selector.lvclass">)
            n64 = Increment(x=w193) -> (x+1=w192:i32)
            n65 = call <vilib>:"Add State(s) to Queue__jki_lib_state_machine.vi"("State(s) in Front (\"\")"="MCLB: Reorder\nIntegration: Insert Subpanel\nIntegration: Set Active", "State(s) in (\"\")"=w200) -> ("States Out"=w199:string)  [unwired: 13 in]
          }
          event "Multicolumn Listbox": Drag Starting {
            # "Timeout Frame\n(this will only execute if the Event Structure timeout is >= 0)"
            n66 = event-data() -> ()  [unwired: 1 in, 10 out]
            n67 = call <vilib>:"Add State(s) to Queue__jki_lib_state_machine.vi"("State(s) in (\"\")"=w206) -> ("States Out"=w205:string)  [unwired: 14 in]
          }
          event "Multicolumn Listbox": Drag Ended {
            # "Timeout Frame\n(this will only execute if the Event Structure timeout is >= 0)"
            n68 = event-data() -> ("CtlRef"=w215:refnum<vi>)  [unwired: 1 in, 4 out]
            n69 = property class="MCListbox (strict)"(reference=w215) -> ("ItemNames"=w214:string[][], "Value"=w208:i32)  [unwired: 1 in, 2 out]
            n70 = Bundle By Name(cluster=w211, "Item Names"=w214) -> (w212:T19)
            n71 = Bundle By Name(cluster=w209, "Value"=w208) -> (w210:refnum<class "Selector.lvclass">)
            n72 = Increment(x=w208) -> (x+1=w207:i32)
            n73 = call <vilib>:"Add State(s) to Queue__jki_lib_state_machine.vi"("State(s) in Front (\"\")"="MCLB: Reorder\n//Integration: Insert Subpanel\nMCLB: Order Litho Data", "State(s) in (\"\")"=w219) -> ("States Out"=w218:string)  [unwired: 13 in]
          }
          event "Multicolumn Listbox": Shortcut Menu Selection (User) {
            # "Timeout Frame\n(this will only execute if the Event Structure timeout is >= 0)"
            n74 = event-data() -> ("ItemPath"=w226:string)  [unwired: 1 in, 7 out]
            n75 = Match Pattern(string=w226, regular expression="\\:") -> (before substring=w222:string)  [unwired: 1 in, 3 out]
            n76 = Bundle By Name(cluster=w224, "menu path"=w226) -> (w225:T19)
            n77 = call <vilib>:"Build State String with Arguments__JKI_lib_State_Machine.vi"("Arguments (\"\")"=w222, "State"="MCLB: SCM Selection") -> ("State with Arguments"=w221:string)  [unwired: 4 in]
            n78 = call <vilib>:"Add State(s) to Queue__jki_lib_state_machine.vi"("State(s) in Front (\"\")"=w221, "State(s) in (\"\")"=w231) -> ("States Out"=w230:string)  [unwired: 13 in]
          }
          event "Multicolumn Listbox": Shortcut Menu Activation? {
            # "Timeout Frame\n(this will only execute if the Event Structure timeout is >= 0)"
            n79 = event-data() -> ("MenuRef"=w238:refnum<k9>, "Coords"=w237:T20)  [unwired: 1 in, 5 out]
            n80 = call-dynamic "Populate Menu Activation.vi"("error in (no error)"=w234, "Point32"=w237, "MenuRef"=w238, "Selector in"=w232) -> ("error out"=w235:errorcluster, "Selector out"=w239:refnum<class "Selector.lvclass">)  [unwired: 6 in]
            n81 = event-data("Discard?"=FALSE) -> ()  [unwired: 1 in, 1 out]
            n82 = call <vilib>:"Add State(s) to Queue__jki_lib_state_machine.vi"("State(s) in (\"\")"=w242) -> ("States Out"=w241:string)  [unwired: 14 in]
          }
          event "Multicolumn Listbox": Mouse Down? {
            # "Timeout Frame\n(this will only execute if the Event Structure timeout is >= 0)"
            n83 = event-data() -> ("Coords"=w254:T20, "Button"=w253:u16, "PlatMods"=w255:T21)  [unwired: 1 in]
            n84 = Bundle By Name(cluster=T6 {"Point"={"Left"=0, "Top"=0}, "Button"=0, "PlatMods"={"Shift"=FALSE, "Ctrl"=FALSE, "Alt"=FALSE, "Cmd"=FALSE, "Opt"=FALSE}} ("Event Data"), "Point"=w254, "Button"=w253, "PlatMods"=w255) -> (w247:T6)
            n85 = call-dynamic "Handle Mouse Down.vi"("error in (no error)"=w257, "Event Data"=w247, "Selector in"=w258) -> ("error out"=w252:errorcluster, "Enable Change"=w246:bool, "Selector out"=w250:refnum<class "Selector.lvclass">)  [unwired: 6 in]
            n86 = case shown="False" w246 {
              tunnel: w250 -> [w263 w267]
              tunnel: w252 -> [w262 w266]
              tunnel: [w262 w265] -> w251
              tunnel: [w263 w264] -> w249
              frame False {
              }
              frame True {
                n87 = call "Change Active Enable Symbol.vi"("error in (no error)"=w266, "Selector in"=w267) -> ("error out"=w265:errorcluster, "Selector out"=w264:refnum<class "Selector.lvclass">)  [unwired: 7 in, 1 out]
              }
            }
            n88 = Select(t="Integration: Change Enable", s=w246, f="") -> (s? t:f=w245:string)
            n89 = event-data("Discard?"=w246) -> ()  [unwired: 1 in, 1 out]
            n90 = call <vilib>:"Add State(s) to Queue__jki_lib_state_machine.vi"("State(s) in Front (\"\")"=w245, "State(s) in (\"\")"=w261) -> ("States Out"=w260:string)  [unwired: 13 in]
          }
          event Panel Close? {
            # "Discard the event because we'll close the front panel ourselves in Macro: Exit"
            # "Close Panel button (pressed) Event\n(this executes Macro: Exit to terminate the VI)"
            n91 = event-data() -> ()  [unwired: 1 in, 1 out]
            n92 = event-data("Discard?"=TRUE) -> ()  [unwired: 1 in, 1 out]
            n93 = call <vilib>:"Add State(s) to Queue__jki_lib_state_machine.vi"("State(s) in Front (\"\")"="Macro: Exit", "State(s) in (\"\")"=w274) -> ("States Out"=w273:string)  [unwired: 13 in]
          }
        }
      }
      frame "---------- Core ----------" {
        # "Do not put any code in this frame.\n(it is a separator no-op)"
        n94 = call <vilib>:"Add State(s) to Queue__jki_lib_state_machine.vi"("State(s) in (\"\")"=w280) -> ("States Out"=w279:string)  [unwired: 14 in]
      }
      frame Default {
        w292 = 42 items=["No error", "Argument error", "Memory is full", "Out of zone", "End of file", "File already open", "Generic file I/O error", "File not found", "File permission error", "Disk is full", "Duplicate path", "Too many files open", "System feature not enabled", "Resource file not found", "Cannot add resource", "Resource not found", "Image not found", "Image memory error", "Pen does not exist", "Config type invalid", "Config token not found", "Config parse error", "Config memory error", "Bad external code format", "Bad external code offset", "External code not present", "Null window", "Destroy window error", "Null menu", "Print aborted", "Bad print record", "Print driver error", "Windows error during printing", "Memory error during printing", "Print dialog error", "Generic print error", "Invalid device refnum", "Device not found", "Device parameter error", "Device unit error", "Cannot open device", "Device call aborted", "Generic error", "Cancelled by user", "Object ID too low", "Object ID too high", "Object not in heap", "Unknown heap", "Unknown object (invalid DefProc)", "Unknown object (DefProc not in table)", "Message out of range", "Invalid (null) method", "Unknown message", "Manager call not supported", "Bad address", "Network operation in progress", "Network operation timed out", "Connection is busy", "Network attribute not supported", "Network error", "Address in use", "System out of memory", "Connection aborted", "Connection refused", "Not connected", "Already connected", "Connection closed", "Initialization error (interapplication manager)", "Bad occurrence", "Wait on unbound occurrence handler", "Occurrence queue overflow", "Datalog type conflict", "Unused", "Unrecognized type (interapplication manager)", "Memory corrupt", "Failed to make temporary DLL", "Old CIN version", "Drag socket not found", "Failed to load drop-object", "Failed to register OLE object", "Failed to release OLE object", "Format specifier type mismatch", "Unknown format specifier", "Too few format specifiers", "Too many format specifiers", "Scan failed", "Newer CIN version", "Error converting to variant", "Runtime menu error", "Password tampered", "Variant attribute not found", "Incompatible variant data type", "Event data is not available", "Event Store is not present", "Occurrence is not found", "Event Queue is not created", "Event info is not available", "Refnum passed is NULL", "Error retrieving Class GUID", "Error retrieving CoClass GUID", "Error retrieving TypeLib GUID.", "Bad built application magic bytes.", "Specific driver is different from the specific driver associated with the Logical Name.", "There is no session opened to the class driver.", "Max Error", "MAX - Error with config objects", "MAX - Error loading configuration", "MAX - Group not supported"]
        # "State Syntax:\nStateCategory: State >> Argument\nLine Terminator: Line feed\nExample:\nUI: Help >> About\n\nWhere \"UI\" is the state category\nWhere \"Help\" is the state\nWhere \"About\" is the argument\nOther Examples:\nApp Data: Initialize\nUI: Initialize\nHelp >> About\n\nCommenting:\nTo add a comment use \"//\" or \"#\" and all text to the right will be ignored\nCommenting Example:\nUI: Initialize // This initializes the UI\n# This whole line is a comment\n// Another comment line"
        # "Current State"
        # "Do not delete, rename, or modify this frame.\n(this is used to capture unhandled states and typos)"
        # "Handle mistyped state name (developer tool)"
        n95 = Format Into String(format string="Software Exception: Unhandled State \"%s\"." ("message"), error in=w288, w283) -> (resulting string=w291:string, error out=w290:errorcluster)  [unwired: 1 in]
        n96 = call <vilib>:"Error Cluster From Error Code.vi"("show call chain? (False)"=TRUE, "error in (no error)"=w290, "error message (\"\")"=w291, "error code (0)"=w292) -> ("error out"=w289:errorcluster)  [unwired: 5 in]
        n97 = call <vilib>:"Add State(s) to Queue__jki_lib_state_machine.vi"("State(s) in (\"\")"=w287) -> ("States Out"=w286:string)  [unwired: 14 in]
      }
      frame "Initialize Core Data" {
        # "Do not delete, rename, or modify this frame.\n(this is used to determine panel behavior on exit)"
        # "originally closed?"
        # "exe?"
        # "If panel starts closed or is an EXE, then close it when we exit"
        n98 = property class="VI"() -> ("FP.State"=w298:T7)  [unwired: 2 in, 2 out]
        n99 = property class="App"() -> ("App.Kind"=w304:T8)  [unwired: 2 in, 2 out]
        n100 = control-ref of="Current VI Reference"() -> (w299:refnum<vi>)
        n101 = Equal?(x=w298, y=T7."Closed" ("Front Panel Window:State")) -> (x = y?=w296:bool)
        n102 = Equal?(x=w304, y=T8."Run Time System" ("Application:Kind")) -> (x = y?=w302:bool)
        n103 = Or(x=w296, y=w302) -> (x .or. y?=w300:bool)
        n104 = Bundle By Name(cluster=w301, "Core.Current VI Reference"=w299, "Core.Close Panel on Exit?"=w300) -> (w306:T19)
        n105 = call <vilib>:"Add State(s) to Queue__jki_lib_state_machine.vi"("State(s) in (\"\")"=w308) -> ("States Out"=w307:string)  [unwired: 14 in]
      }
      frame "Error Handler" {
        # "Unhandled Error -- Display it"
        # "Handle any errors here.\nYou can also output any states to clean-up after errors occur"
        # "Clear error"
        n106 = call <vilib>:"General Error Handler.vi"("error in (no error)"=w312) -> ()  [unwired: 10 in, 5 out]
        n107 = call <vilib>:"Add State(s) to Queue__jki_lib_state_machine.vi"("State(s) in Front (\"\")"="/* Post Error States", "State(s) in (\"\")"=w316) -> ("States Out"=w315:string)  [unwired: 13 in]
      }
      frame "Exit" {
        # "Do not put any code in this frame.\n(No errors that occur here will be handled.)"
        n108 = call <vilib>:"Add State(s) to Queue__jki_lib_state_machine.vi"("State(s) in (\"\")"=w323) -> ("States Out"=w322:string)  [unwired: 14 in]
      }
      frame "---------- Data ----------" {
        # "Do not put any code in this frame.\n(It is a separator no-op. You can make a copy of this frame to create a new Data frame)"
        n109 = call <vilib>:"Add State(s) to Queue__jki_lib_state_machine.vi"("State(s) in (\"\")"=w329) -> ("States Out"=w328:string)  [unwired: 14 in]
      }
      frame "Data: Initialize MCLB" {
        # "Do not put any code in this frame.\n(It is a separator no-op. You can make a copy of this frame to create a new Data frame)"
        n110 = control-ref of="Multicolumn Listbox"() -> (w332:refnum<vi>)
        n111 = property class="MCListbox (strict)"(reference=w332) -> (reference out=w333:refnum<vi>, "ItemNames"=w337:string[][], "ItemSyms"=w336:i32[])  [unwired: 1 in, 1 out]
        n112 = Greater Than 0?(x=w336) -> (x > 0?=w335:bool[])
        n113 = for {
          tunnel: w335 -> [w345] mode=indexing
          tunnel: [w344] -> w334 mode=indexing
          tunnel: w337 -> [w343] mode=indexing
          n114 = Index Array(array=w343) -> (element #1=w347:string, element #2=w346:string)  [unwired: 2 in]
          n115 = Bundle By Name(cluster=T9 {"Name"="", "Group"="", "Enabled"=FALSE} ("Item"), "Name"=w347, "Group"=w346, "Enabled"=w345) -> (w344:T9)
        }
        n116 = Bundle By Name(cluster=w330, "Reference"=w333, "Item Names"=w337, "Enabled"=w335, "Items"=w334) -> (w331:refnum<class "Selector.lvclass">)
        n117 = call <vilib>:"Add State(s) to Queue__jki_lib_state_machine.vi"("State(s) in (\"\")"=w342) -> ("States Out"=w341:string)  [unwired: 14 in]
      }
      frame "Data: Initialize" {
        w360 = T22 {"Path Changes"=[], "Funnel Changes"=[], "Rectangle Changes"=[], "Dot Changes"=[]}  # Changed Objects
        w358 = T4 []  # Lithography Data
        w357 = T23 {"Rectangles"=[], "Paths"=[], "Funnels"=[], "Dots"=[]}  # Obj Settings
        w354 = T24 {"Dots"=[], "Funnels"=[], "Rects"=[], "Paths"=[]}  # GUIDs
        w353 = T25 {"Paths"=[], "Rectangles"=[], "SVGImage"=refnum, "Dots"=[], "Funnels"=[]}  # Parsed Data
        w359 = refnum<class "BigMAQ.lvclass"> refnum  # BigMAQ
        w356 = refnum<class "Tool Data.lvclass"> refnum  # Tooler
        w355 = refnum<class "Subpanel.Edit.lvclass"> refnum  # Subpanel.Edit
        w351 = refnum<class "Setting Database.lvclass"> refnum  # Settings
        w352 = refnum<class "ParseVectorFile.lvclass"> refnum  # Parser
        w350 = string[][] []  # Item Names
        w349 = ""  # menu path
        w364 = T26 {"Current VI Reference"=refnum, "Close Panel on Exit?"=FALSE}  # Core
        # "do not delete - used by framework"
        # "Data names and types of shift register data are defined by this bundle."
        # "Initialize the shift-register data, here.\n(data names are defined by what you wire into the bundle function)"
        n118 = Bundle("Core"=w364, "menu path"=w349, "Item Names"=w350, "Settings"=w351, "Parser"=w352, "Parsed Data"=w353, "GUIDs"=w354, "Subpanel.Edit"=w355, "Tooler"=w356, "Obj Settings"=w357, "Lithography Data"=w358, "BigMAQ"=w359, "Changed Objects"=w360) -> (w365:T19)  [unwired: 1 in]
        n119 = call <vilib>:"Add State(s) to Queue__jki_lib_state_machine.vi"("State(s) in (\"\")"=w367) -> ("States Out"=w366:string)  [unwired: 14 in]
      }
      frame "Data: Cleanup" {
        # "Cleanup any data and references, here.\n(this is called automatically, by the Macro: Exit)"
        n120 = Unbundle By Name(w373) -> ("Core.Current VI Reference"=w375:refnum<vi>, "BigMAQ"=w370:refnum<class "BigMAQ.lvclass">)
        n121 = call <vilib>:"Destroy.vi"("error in"=w368, "BigMAQ in"=w370) -> ("error out"=w369:errorcluster)  [unwired: 8 in, 1 out]
        n122 = Close Reference(reference=w375, error in (no error)=w369) -> (error out=w374:errorcluster)
        n123 = call <vilib>:"Add State(s) to Queue__jki_lib_state_machine.vi"("State(s) in (\"\")"=w377) -> ("States Out"=w376:string)  [unwired: 14 in]
      }
      frame "---------- Events ----------" {
        # "Do not put any code in this frame.\n(It is a separator no-op. You can make a copy of this frame to create a new UI frame)"
        n124 = call <vilib>:"Add State(s) to Queue__jki_lib_state_machine.vi"("State(s) in (\"\")"=w383) -> ("States Out"=w382:string)  [unwired: 14 in]
      }
      frame "Events: Register" {
        # "Do not put any code in this frame.\n(It is a separator no-op. You can make a copy of this frame to create a new UI frame)"
        n125 = Unbundle By Name(w395) -> ("Settings"=w394:refnum<class "Setting Database.lvclass">, "Parser"=w392:refnum<class "ParseVectorFile.lvclass">, "Tooler"=w386:refnum<class "Tool Data.lvclass">)
        n126 = call "Tool Data.GetPublicEvents.vi"("Tool Data"=w386) -> ("error out"=w384:errorcluster, "Public Events"=w385:T27)  [unwired: 8 in, 1 out]
        n127 = call "ParseVectorFile.GetPublicEvents.vi"("error in (no error)"=w390, "ParseVectorFile"=w392) -> ("error out"=w387:errorcluster, "Public Events"=w391:T28)  [unwired: 7 in, 1 out]
        n128 = call "Setting Database.GetPublicEvents.vi"("error in (no error)"=w390, "Setting Database"=w394) -> ("error out"=w388:errorcluster, "Public Events"=w393:T29)  [unwired: 7 in, 1 out]
        n129 = register-events(error in=w390, w393, w391, w385) -> (reference out=w397:refnum<event-registration>, error out=w396:errorcluster)  [unwired: 1 in]
        n130 = Merge Errors(w384, w388, w387, w396) -> (w389:errorcluster)
        n131 = call <vilib>:"Add State(s) to Queue__jki_lib_state_machine.vi"("State(s) in (\"\")"=w400) -> ("States Out"=w399:string)  [unwired: 14 in]
      }
      frame "Events: Unregister" {
        # "Do not put any code in this frame.\n(It is a separator no-op. You can make a copy of this frame to create a new UI frame)"
        n132 = Unregister For Events(event registration refnum=w403, error in=w402) -> (error out=w401:errorcluster)
        n133 = call <vilib>:"Add State(s) to Queue__jki_lib_state_machine.vi"("State(s) in (\"\")"=w407) -> ("States Out"=w406:string)  [unwired: 14 in]
      }
      frame "---------- UI ----------" {
        # "Do not put any code in this frame.\n(It is a separator no-op. You can make a copy of this frame to create a new UI frame)"
        n134 = call <vilib>:"Add State(s) to Queue__jki_lib_state_machine.vi"("State(s) in (\"\")"=w413) -> ("States Out"=w412:string)  [unwired: 14 in]
      }
      frame "UI: Update MCLB" {
        # "Do not put any code in this frame.\n(It is a separator no-op. You can make a copy of this frame to create a new UI frame)"
        n135 = Unbundle By Name(w419) -> ("Reference"=w417:refnum<vi>, "Items"=w418:T30[])
        n136 = call "Items to MCLB Item Names.vi"("Items"=w418) -> ("Item Names"=w416:string[][])  [unwired: 6 in]
        n137 = property class="MCListbox"(reference=w417, error in=w414, "ItemNames"=w416) -> (error out=w415:errorcluster)  [unwired: 1 out]
        n138 = call <vilib>:"Add State(s) to Queue__jki_lib_state_machine.vi"("State(s) in (\"\")"=w423) -> ("States Out"=w422:string)  [unwired: 14 in]
      }
      frame "UI: Initialize" {
        # "Initialize the User Interface, here.\n(this is called automatically, by the Macro: Init)"
        n139 = control-ref of="Render"() -> (w424:refnum<vi>)
        n140 = call <vilib>:"Create.vi"("error in (no error)"=w432, "Resolution"=1024, "Reference"=w424) -> ("error out"=w431:errorcluster, "To Control"=→"Render":T1, "BigMAQ out"=w428:refnum<class "BigMAQ.lvclass">)  [unwired: 6 in]
        n141 = call-dynamic "Initialize Control Appearance.vi"("error in (no error)"=w431, "Selector in"=w439) -> ("error out"=w437:errorcluster, "Selector out"=w436:refnum<class "Selector.lvclass">)  [unwired: 8 in]
        n142 = call-dynamic "Setup Item Symbols.vi"("error in (no error)"=w437, "Selector in"=w436) -> ("error out"=w426:errorcluster, "Selector out"=w435:refnum<class "Selector.lvclass">)  [unwired: 8 in]
        n143 = call "Initialize UI.vi"("error in"=w426, "BigMAQ in"=w428) -> ("error out"=w425:errorcluster, "BigMAQ out"=w427:refnum<class "BigMAQ.lvclass">)  [unwired: 8 in]
        n144 = Bundle By Name(cluster=w433, "BigMAQ"=w427) -> (w434:T19)
        n145 = call <vilib>:"Add State(s) to Queue__jki_lib_state_machine.vi"("State(s) in (\"\")"=w441) -> ("States Out"=w440:string)  [unwired: 14 in]
      }
      frame "UI: Cursor Set" {
        # "Argument"
        # "Set and Unset Cursor Busy.\n(Usage: \"UI: Cursor Set >> Busy|Idle\")"
        n146 = case shown="\"Idle\", Default" w444 {
          tunnel: w446 -> [w451 w453]
          tunnel: [w450 w452] -> w445
          frame "Idle", Default {
            n147 = call <vilib>:"Unset Busy.vi"("error in (no error)"=w451) -> ("error out"=w450:errorcluster)  [unwired: 10 in]
          }
          frame "Busy" {
            n148 = call <vilib>:"Set Busy.vi"("error in (no error)"=w453) -> ("error out"=w452:errorcluster)  [unwired: 9 in, 1 out]
          }
        }
        n149 = call <vilib>:"Add State(s) to Queue__jki_lib_state_machine.vi"("State(s) in (\"\")"=w449) -> ("States Out"=w448:string)  [unwired: 14 in]
      }
      frame "UI: Front Panel State" {
        # "Argument"
        # "Set Front Panel Open or Closed\n(Usage: \"UI: Front Panel State >> Open|Close\")"
        n150 = Unbundle By Name(w458) -> ("Core.Current VI Reference"=w457:refnum<vi>)
        n151 = case shown="\"Minimize\", \"Minimized\"" w456 {
          tunnel: w460 -> [w468 w483 w494 w507 w520]
          tunnel: [w470 w484 w496 w509 w522] -> w459
          tunnel: w457 -> [w469 w481 w495 w508 w521]
          frame "Open", "Standard", Default {
            w463 = T7."Standard" ("State")
            n152 = property class="VI"(reference=w469, error in=w468) -> (reference out=w466:refnum<vi>, error out=w467:errorcluster, "FP.State"=w465:T7)
            n153 = Not Equal?(x=w465, y=w463) -> (x != y?=w464:bool)
            n154 = case shown="True" w464 {
              tunnel: [w474 w476] -> w470
              tunnel: w467 -> [w473 w476]
              tunnel: w466 -> [w472 _]
              tunnel: w463 -> [w471 _]
              frame True {
                n155 = invoke class="VI" method="FP.Open"(reference=w472, error in=w473, "Activate"=TRUE, "State"=w471) -> (error out=w474:errorcluster)  [unwired: 1 in, 4 out]
              }
              frame False {
              }
            }
          }
          frame "Close", "Closed" {
            n156 = property class="VI"(reference=w481, error in=w483) -> (reference out=w480:refnum<vi>, error out=w482:errorcluster, "FP.State"=w478:T7)
            n157 = Not Equal?(x=w478, y=T7."Closed" ("Front Panel Window:State")) -> (x != y?=w477:bool)
            n158 = case shown="True" w477 {
              tunnel: [w485 w488] -> w484
              tunnel: w482 -> [w485 w487]
              tunnel: w480 -> [_ w486]
              frame False {
              }
              frame True {
                n159 = invoke class="VI" method="FP.Close"(reference=w486, error in=w487) -> (error out=w488:errorcluster)  [unwired: 1 in, 2 out]
              }
            }
          }
          frame "Hidden", "Hide" {
            w489 = T7."Hidden" ("State")
            n160 = property class="VI"(reference=w495, error in=w494) -> (reference out=w492:refnum<vi>, error out=w493:errorcluster, "FP.State"=w491:T7)
            n161 = Not Equal?(x=w491, y=w489) -> (x != y?=w490:bool)
            n162 = case shown="True" w490 {
              tunnel: [w500 w501] -> w496
              tunnel: w493 -> [w499 w501]
              tunnel: w492 -> [w498 _]
              tunnel: w489 -> [w497 _]
              frame True {
                n163 = invoke class="VI" method="FP.Open"(reference=w498, error in=w499, "State"=w497) -> (error out=w500:errorcluster)  [unwired: 2 in, 4 out]
              }
              frame False {
              }
            }
          }
          frame "Minimize", "Minimized" {
            w502 = T7."Minimized" ("State")
            n164 = property class="VI"(reference=w508, error in=w507) -> (reference out=w505:refnum<vi>, error out=w506:errorcluster, "FP.State"=w504:T7)
            n165 = Not Equal?(x=w504, y=w502) -> (x != y?=w503:bool)
            n166 = case shown="True" w503 {
              tunnel: [w513 w514] -> w509
              tunnel: w506 -> [w512 w514]
              tunnel: w505 -> [w511 _]
              tunnel: w502 -> [w510 _]
              frame True {
                n167 = invoke class="VI" method="FP.Open"(reference=w511, error in=w512, "State"=w510) -> (error out=w513:errorcluster)  [unwired: 2 in, 4 out]
              }
              frame False {
              }
            }
          }
          frame "Maximize", "Maximized" {
            w515 = T7."Maximized" ("State")
            n168 = property class="VI"(reference=w521, error in=w520) -> (reference out=w518:refnum<vi>, error out=w519:errorcluster, "FP.State"=w517:T7)
            n169 = Not Equal?(x=w517, y=w515) -> (x != y?=w516:bool)
            n170 = case shown="True" w516 {
              tunnel: [w526 w527] -> w522
              tunnel: w519 -> [w525 w527]
              tunnel: w518 -> [w524 _]
              tunnel: w515 -> [w523 _]
              frame True {
                n171 = invoke class="VI" method="FP.Open"(reference=w524, error in=w525, "State"=w523) -> (error out=w526:errorcluster)  [unwired: 2 in, 4 out]
              }
              frame False {
              }
            }
          }
        }
        n172 = call <vilib>:"Add State(s) to Queue__jki_lib_state_machine.vi"("State(s) in (\"\")"=w462) -> ("States Out"=w461:string)  [unwired: 14 in]
      }
      frame "UI: MCLB Symbols" {
        # "Your code here.\n(You can make a copy of, or modify, this frame)"
        n173 = call-dynamic "Apply Item Symbols.vi"("error in (no error)"=w529, "Selector in"=w530) -> ("error out"=w528:errorcluster, "Selector out"=w532:refnum<class "Selector.lvclass">)  [unwired: 8 in]
        n174 = call <vilib>:"Add State(s) to Queue__jki_lib_state_machine.vi"("State(s) in (\"\")"=w535) -> ("States Out"=w534:string)  [unwired: 14 in]
      }
      frame "---------- Macro ----------" {
        # "Do not put any code in this frame.\n(It is a separator no-op. You can make a copy of this frame to create a new Macro frame)"
        n175 = call <vilib>:"Add State(s) to Queue__jki_lib_state_machine.vi"("State(s) in (\"\")"=w541) -> ("States Out"=w540:string)  [unwired: 14 in]
      }
      frame "Macro: Initialize" {
        # "Initialization Macro\n(This is called once, when the VI starts)"
        n176 = call <vilib>:"Add State(s) to Queue__jki_lib_state_machine.vi"("State(s) in Front (\"\")"="Data: Initialize\nInitialize Core Data\nData: Initialize MCLB\nIntegration: Start SMOs\nEvents: Register\nIntegration: Parser SVG\nUI: Initialize\nIntegration: Read IBW\nIntegration: Update BigMAQ\nUI: Front Panel State >> Open\nUI: MCLB Symbols\n", "State(s) in (\"\")"=w548) -> ("States Out"=w547:string)  [unwired: 13 in]
      }
      frame "Macro: Exit" {
        # "Exit Macro\n(This is called once, when the VI exits)"
        n177 = Unbundle By Name(w557) -> ("Core.Close Panel on Exit?"=w556:bool)
        n178 = Select(t="UI: Front Panel State >> Close", s=w556, f="") -> (s? t:f=w553:string)
        n179 = call <vilib>:"Add State(s) to Queue__jki_lib_state_machine.vi"("State(s) in (\"\")"=w553, "State(s) at Back (\"\")"="Data: Cleanup\nIntegration: Stop SMOs\nEvents: Unregister\nExit") -> ("States Out"=w551:string)  [unwired: 13 in]
        n180 = call <vilib>:"Add State(s) to Queue__jki_lib_state_machine.vi"("State(s) in Front (\"\")"=w551, "State(s) in (\"\")"=w560) -> ("States Out"=w559:string)  [unwired: 13 in]
      }
      frame "---------- Integration ----------" {
        # "Template Separator\n(You can make a copy of, or modify, this frame)"
        n181 = Unbundle By Name(w566) -> ("Settings"=w565:refnum<class "Setting Database.lvclass">, "Parser"=w564:refnum<class "ParseVectorFile.lvclass">, "Tooler"=w563:refnum<class "Tool Data.lvclass">, "BigMAQ"=w562:refnum<class "BigMAQ.lvclass">)
        n182 = Bundle By Name(cluster=w566, "Settings"=w565, "Parser"=w564, "Tooler"=w563, "BigMAQ"=w562) -> (w567:T19)
        n183 = call <vilib>:"Add State(s) to Queue__jki_lib_state_machine.vi"("State(s) in (\"\")"=w571) -> ("States Out"=w570:string)  [unwired: 14 in]
      }
      frame "Integration: Specific Overlays" {
        # "Template Separator\n(You can make a copy of, or modify, this frame)"
        n184 = Unbundle By Name(w585) -> ("Settings"=w584:refnum<class "Setting Database.lvclass">, "Parser"=w583:refnum<class "ParseVectorFile.lvclass">, "Tooler"=w582:refnum<class "Tool Data.lvclass">, "BigMAQ"=w575:refnum<class "BigMAQ.lvclass">, "Changed Objects"=w580:T22, "Lithography Data"=w572:T4)
        n185 = Unbundle By Name(w580) -> ("Path Changes"=w579:cluster{bool, "index of element":i32}[], "Funnel Changes"=w578:cluster{bool, "index of element":i32}[], "Rectangle Changes"=w577:cluster{bool, "index of element":i32}[], "Dot Changes"=w576:cluster{bool, "index of element":i32}[])
        n186 = Build Array (concatenate)(w579, w578, w577, w576) -> (w573:cluster{bool, "index of element":i32}[])
        n187 = for {
          shift-right: [w594] -> w574
          shift-left: w575 -> [w595]
          tunnel: w573 -> [w593] mode=indexing
          tunnel: w572 -> [w591] mode=indexing
          n188 = Unbundle(w593) -> (w592:bool)  [unwired: 1 out]
          n189 = case shown="True" w592 {
            tunnel: w595 -> [w596 w600]
            tunnel: [w596 w599] -> w594
            tunnel: w591 -> [_ w598]
            frame False {
            }
            frame True {
              n190 = call "Replace Single Overlay.vi"("Show Text"=TRUE, "Litho"=w598, "BigMAQ in"=w600) -> ("BigMAQ out"=w599:refnum<class "BigMAQ.lvclass">)  [unwired: 7 in, 1 out]
            }
          }
        }
        n191 = Bundle By Name(cluster=w585, "Settings"=w584, "Parser"=w583, "Tooler"=w582, "BigMAQ"=w574) -> (w586:T19)
        n192 = call <vilib>:"Add State(s) to Queue__jki_lib_state_machine.vi"("State(s) in (\"\")"=w590) -> ("States Out"=w589:string)  [unwired: 14 in]
      }
      frame "Integration: Zoom to Fit" {
        # "Template Separator\n(You can make a copy of, or modify, this frame)"
        n193 = Unbundle By Name(w608) -> ("Settings"=w607:refnum<class "Setting Database.lvclass">, "Parser"=w606:refnum<class "ParseVectorFile.lvclass">, "Tooler"=w605:refnum<class "Tool Data.lvclass">, "BigMAQ"=w604:refnum<class "BigMAQ.lvclass">)
        n194 = call "Zoom to Fit.vi"("error in"=w601, "BigMAQ in"=w604) -> ("error out"=w602:errorcluster, "BigMAQ out"=w603:refnum<class "BigMAQ.lvclass">)  [unwired: 7 in, 1 out]
        n195 = Bundle By Name(cluster=w608, "Settings"=w607, "Parser"=w606, "Tooler"=w605, "BigMAQ"=w603) -> (w609:T19)
        n196 = call <vilib>:"Add State(s) to Queue__jki_lib_state_machine.vi"("State(s) in (\"\")"=w613) -> ("States Out"=w612:string)  [unwired: 14 in]
      }
      frame "Integration: Overlay" {
        # "Template Separator\n(You can make a copy of, or modify, this frame)"
        n197 = Unbundle By Name(w623) -> ("Settings"=w622:refnum<class "Setting Database.lvclass">, "Parser"=w621:refnum<class "ParseVectorFile.lvclass">, "Tooler"=w620:refnum<class "Tool Data.lvclass">, "BigMAQ"=w619:refnum<class "BigMAQ.lvclass">, "Lithography Data"=w617:T4)
        n198 = call "Generate New Overlay.vi"("Label?"=TRUE, "error in"=w615, "Lithography Data"=w617, "BigMAQ in"=w619) -> ("error out"=w616:errorcluster, "BigMAQ out"=w618:refnum<class "BigMAQ.lvclass">)  [unwired: 6 in]
        n199 = Bundle By Name(cluster=w623, "Settings"=w622, "Parser"=w621, "Tooler"=w620, "BigMAQ"=w618) -> (w624:T19)
        n200 = call <vilib>:"Add State(s) to Queue__jki_lib_state_machine.vi"("State(s) in (\"\")"=w628) -> ("States Out"=w627:string)  [unwired: 14 in]
      }
      frame "Integration: Update BigMAQ" {
        # "Template Separator\n(You can make a copy of, or modify, this frame)"
        n201 = Unbundle By Name(w636) -> ("Settings"=w635:refnum<class "Setting Database.lvclass">, "Parser"=w634:refnum<class "ParseVectorFile.lvclass">, "Tooler"=w633:refnum<class "Tool Data.lvclass">, "BigMAQ"=w632:refnum<class "BigMAQ.lvclass">)
        n202 = call "Update Control.vi"("error in"=w629, "BigMAQ in"=w632) -> ("error out"=w630:errorcluster, "BigMAQ out"=w631:refnum<class "BigMAQ.lvclass">)  [unwired: 8 in]
        n203 = Bundle By Name(cluster=w636, "Settings"=w635, "Parser"=w634, "Tooler"=w633, "BigMAQ"=w631) -> (w637:T19)
        n204 = call <vilib>:"Add State(s) to Queue__jki_lib_state_machine.vi"("State(s) in (\"\")"=w641) -> ("States Out"=w640:string)  [unwired: 14 in]
      }
      frame "Integration: Read IBW" {
        # "Template Separator\n(You can make a copy of, or modify, this frame)"
        n205 = Unbundle By Name(w653) -> ("Settings"=w652:refnum<class "Setting Database.lvclass">, "Parser"=w651:refnum<class "ParseVectorFile.lvclass">, "Tooler"=w650:refnum<class "Tool Data.lvclass">, "BigMAQ"=w649:refnum<class "BigMAQ.lvclass">)
        n206 = call "Read Background.vi"("error in (no error)"=w647, "Path"="IBW", "BigMAQ in"=w649) -> ("error out"=w643:errorcluster, "BigMAQ out"=w646:refnum<class "BigMAQ.lvclass">)  [unwired: 6 in, 1 out]
        n207 = call-dynamic "Write Size.vi"("error in (no error)"=w643, "Size"=40.0, "BigMAQ in"=w646) -> ("error out"=w642:errorcluster, "BigMAQ out"=w645:refnum<class "BigMAQ.lvclass">)  [unwired: 7 in]
        n208 = Bundle By Name(cluster=w653, "Settings"=w652, "Parser"=w651, "Tooler"=w650, "BigMAQ"=w645) -> (w654:T19)
        n209 = call <vilib>:"Add State(s) to Queue__jki_lib_state_machine.vi"("State(s) in (\"\")"=w658) -> ("States Out"=w657:string)  [unwired: 14 in]
      }
      frame "Integration: Graph Litho Data" {
        # "Template Separator\n(You can make a copy of, or modify, this frame)"
        n210 = Unbundle By Name(w663) -> ("Lithography Data"=w662:T4)
        n211 = for {
          tunnel: w662 -> [w672] mode=indexing
          tunnel: [w670] -> w661 mode=concatenating
          tunnel: [w669] -> w660 mode=concatenating
          n212 = Unbundle By Name(w672) -> ("Litho"=w671:T31)
          n213 = for {
            tunnel: w671 -> [w675] mode=indexing
            tunnel: [w674] -> w670 mode=indexing
            tunnel: [w673] -> w669 mode=indexing
            n214 = Unbundle By Name(w675) -> ("X"=w674:dbl, "Y"=w673:dbl)
          }
        }
        n215 = Build Cluster Array(w661, w660) -> (→"XY Graph":cluster{"X":dbl, "Y":dbl}[])
        n216 = call <vilib>:"Add State(s) to Queue__jki_lib_state_machine.vi"("State(s) in (\"\")"=w668) -> ("States Out"=w667:string)  [unwired: 14 in]
      }
      frame "Integration: Generate Data" {
        # "Template Separator\n(You can make a copy of, or modify, this frame)"
        n217 = Unbundle By Name(w683) -> ("Settings"=w682:refnum<class "Setting Database.lvclass">, "Parser"=w681:refnum<class "ParseVectorFile.lvclass">, "Tooler"=w680:refnum<class "Tool Data.lvclass">)
        n218 = call-dynamic "Generate Lithography Data.vi"("error in (no error)"=w677, "Tool Data in"=w680) -> ("error out"=w678:errorcluster, "Lithography Data"=w676:T4, "Tool Data out"=w679:refnum<class "Tool Data.lvclass">)  [unwired: 7 in]
        "Lithography Data" <- w676
        n219 = Bundle By Name(cluster=w683, "Settings"=w682, "Parser"=w681, "Tooler"=w679, "Lithography Data"=w676) -> (w684:T19)
        n220 = call <vilib>:"Add State(s) to Queue__jki_lib_state_machine.vi"("State(s) in (\"\")"=w688) -> ("States Out"=w687:string)  [unwired: 14 in]
      }
      frame "Integration: Tool Data" {
        # "Template Separator\n(You can make a copy of, or modify, this frame)"
        n221 = Unbundle By Name(w707) -> ("Settings"=w706:refnum<class "Setting Database.lvclass">, "Parser"=w705:refnum<class "ParseVectorFile.lvclass">, "Tooler"=w690:refnum<class "Tool Data.lvclass">, "Obj Settings.Rectangles"=w702:T12, "Obj Settings.Paths"=w697:T11, "Obj Settings.Funnels"=w698:T13, "Obj Settings.Dots"=w699:T14, "Parsed Data.Rectangles"=w701:refnum<class "Rectangle.lvclass">[], "Parsed Data.Dots"=w700:refnum<class "Dot.lvclass">[], "Parsed Data.Funnels"=w694:refnum<class "Path.lvclass">[], "Parsed Data.Paths"=w693:refnum<class "Path.lvclass">[])
        n222 = Build Array (concatenate)(w694, w693) -> (w692:refnum<class "Path.lvclass">[])
        n223 = Bundle By Name(cluster=T10 {"Settings"={"Paths"=[], "Rectangles"=[], "Funnels"=[], "Dots"=[]}, "Data"={"Paths"=[], "Rectangles"=[], "SVGImage"=refnum, "Dots"=[], "Funnels"=[]}} ("Updated Objects"), "Settings.Rectangles"=w702, "Settings.Paths"=w697, "Settings.Funnels"=w698, "Settings.Dots"=w699, "Data.Rectangles"=w701, "Data.Dots"=w700, "Data.Paths"=w692) -> (w691:T10)
        n224 = call-dynamic "Find Changed.vi"("Update Objects"=w691, "Tool Data in"=w690) -> ("Changed Objects"=w689:T22)  [unwired: 7 in, 2 out]
        n225 = call "Tool Data.UpdateObjects.vi"("error in (no error)"=w695, "Updated Objects"=w691, "Tool Data"=w690) -> ("error out"=w696:errorcluster, "Tool Data out"=w704:refnum<class "Tool Data.lvclass">)  [unwired: 7 in]
        n226 = Bundle By Name(cluster=w707, "Settings"=w706, "Parser"=w705, "Tooler"=w704, "Changed Objects"=w689) -> (w708:T19)
        n227 = call <vilib>:"Add State(s) to Queue__jki_lib_state_machine.vi"("State(s) in (\"\")"=w712) -> ("States Out"=w711:string)  [unwired: 14 in]
      }
      frame "Integration: Set Active" {
        # "Template Separator\n(You can make a copy of, or modify, this frame)"
        n228 = Unbundle By Name(w727) -> ("Settings"=w724:refnum<class "Setting Database.lvclass">, "Parser"=w726:refnum<class "ParseVectorFile.lvclass">)
        n229 = Unbundle By Name(w719) -> ("Items"=w721:T30[], "Value"=w722:i32)
        n230 = Index Array(array=w721, index=w722) -> (element=w720:T30)
        n231 = Unbundle By Name(w720) -> ("Name"=w717:string)
        n232 = call "Name To Type.vi"("Name"=w717) -> ("Type"=w713:string)  [unwired: 4 in]
        n233 = call "Query Registry.vi"("error in"=w714, "Name In"=w717) -> ("error out"=w715:errorcluster, "Alias"=w716:string)  [unwired: 6 in, 2 out]
        n234 = call "Name To Index.vi"("Name"=w717) -> ("Index"=w725:i32)  [unwired: 4 in]
        n235 = case shown="\"p\"" w713 {
          tunnel: w724 -> [w733 w738 w743 w748 w752]
          tunnel: [w733 w737 w742 w747 w753] -> w723
          tunnel: w725 -> [_ _ _ _ _]
          tunnel: w715 -> [w732 w735 w741 w746 w751]
          tunnel: [w732 w736 w740 w745 w750] -> w718
          tunnel: w716 -> [_ w734 w739 w744 w749]
          frame Default {
          }
          frame "d" {
            n236 = call "Setting Database.SetActiveDot.vi"("error in (no error)"=w735, "SetActiveDot"=w734, "Setting Database"=w738) -> ("error out"=w736:errorcluster, "Setting Database out"=w737:refnum<class "Setting Database.lvclass">)  [unwired: 7 in]
          }
          frame "f" {
            n237 = call "Setting Database.SetActiveFunnel.vi"("error in (no error)"=w741, "SetActiveFunnel"=w739, "Setting Database"=w743) -> ("error out"=w740:errorcluster, "Setting Database out"=w742:refnum<class "Setting Database.lvclass">)  [unwired: 7 in]
          }
          frame "p" {
            n238 = call "Setting Database.SetActivePath.vi"("error in (no error)"=w746, "SetActivePath"=w744, "Setting Database"=w748) -> ("error out"=w745:errorcluster, "Setting Database out"=w747:refnum<class "Setting Database.lvclass">)  [unwired: 7 in]
          }
          frame "r" {
            n239 = call "Setting Database.SetActiveRectangle.vi"("error in (no error)"=w751, "SetActiveRectangle"=w749, "Setting Database"=w752) -> ("error out"=w750:errorcluster, "Setting Database out"=w753:refnum<class "Setting Database.lvclass">)  [unwired: 7 in]
          }
        }
        n240 = Bundle By Name(cluster=w727, "Settings"=w723, "Parser"=w726) -> (w728:T19)
        n241 = call <vilib>:"Add State(s) to Queue__jki_lib_state_machine.vi"("State(s) in (\"\")"=w731) -> ("States Out"=w730:string)  [unwired: 14 in]
      }
      frame "Integration: Insert Subpanel" {
        # "UI flashing on change to a different type of Object\nIt is because there was an event for rearranging and value change every time there is a drag and drop. I also needed to recheck the order prior to putting the VI in the subpanel when I see a value change"
        # "Template Separator\n(You can make a copy of, or modify, this frame)"
        n242 = Unbundle By Name(w765) -> ("Settings"=w758:refnum<class "Setting Database.lvclass">, "Subpanel.Edit"=w756:refnum<class "Subpanel.Edit.lvclass">)
        n243 = Unbundle By Name(w763) -> ("Items"=w761:T30[], "Value"=w762:i32)
        n244 = Index Array(array=w761, index=w762) -> (element=w760:T30)
        n245 = Unbundle By Name(w760) -> ("Name"=w759:string)
        n246 = call "Name To Type.vi"("Name"=w759) -> ("Type"=w757:string)  [unwired: 4 in]
        n247 = call "Insert Into Subpanel.vi"("error in (no error)"=w755, "Key"=w757, "Subpanel.lvclass"=w756) -> ("error out"=w754:errorcluster, "Subpanel out"=w764:refnum<class "Subpanel.Edit.lvclass">)  [unwired: 7 in]
        n248 = Bundle By Name(cluster=w765, "Settings"=w758, "Subpanel.Edit"=w764) -> (w766:T19)
        n249 = call <vilib>:"Add State(s) to Queue__jki_lib_state_machine.vi"("State(s) in (\"\")"=w769) -> ("States Out"=w768:string)  [unwired: 14 in]
      }
      frame "Integration: Generate GUIDs" {
        # "Template Separator\n(You can make a copy of, or modify, this frame)"
        n250 = Unbundle By Name(w788) -> ("Settings"=w787:refnum<class "Setting Database.lvclass">, "Parser"=w786:refnum<class "ParseVectorFile.lvclass">, "Parsed Data.Paths"=w785:refnum<class "Path.lvclass">[], "Parsed Data.Rectangles"=w784:refnum<class "Rectangle.lvclass">[], "Parsed Data.Funnels"=w783:refnum<class "Path.lvclass">[], "Parsed Data.Dots"=w782:refnum<class "Dot.lvclass">[])
        n251 = for {
          tunnel: w783 -> [w805] mode=indexing
          tunnel: [w804] -> w773 mode=indexing
          tunnel: [w800] -> w780 mode=indexing
          i -> [w801]
          n252 = call-dynamic "Read id.vi"("SVG Object in"=w805) -> ("id"=w804:string)  [unwired: 8 in, 2 out]
          n253 = Number To Decimal String(number=w801) -> (decimal integer string=w803:string)  [unwired: 1 in]
          n254 = Concatenate Strings("f" ("string"), w803) -> (w800:string)
        }
        n255 = for {
          tunnel: w784 -> [w811] mode=indexing
          tunnel: [w810] -> w772 mode=indexing
          tunnel: [w806] -> w779 mode=indexing
          i -> [w807]
          n256 = call-dynamic "Read id.vi"("SVG Object in"=w811) -> ("id"=w810:string)  [unwired: 8 in, 2 out]
          n257 = Number To Decimal String(number=w807) -> (decimal integer string=w809:string)  [unwired: 1 in]
          n258 = Concatenate Strings("r" ("string"), w809) -> (w806:string)
        }
        n259 = for {
          tunnel: w785 -> [w817] mode=indexing
          tunnel: [w816] -> w771 mode=indexing
          tunnel: [w812] -> w778 mode=indexing
          i -> [w815]
          n260 = call-dynamic "Read id.vi"("SVG Object in"=w817) -> ("id"=w816:string)  [unwired: 8 in, 2 out]
          n261 = Number To Decimal String(number=w815) -> (decimal integer string=w814:string)  [unwired: 1 in]
          n262 = Concatenate Strings("p" ("string"), w814) -> (w812:string)
        }
        n263 = for {
          tunnel: w782 -> [w799] mode=indexing
          tunnel: [w798] -> w774 mode=indexing
          tunnel: [w794] -> w781 mode=indexing
          i -> [w795]
          n264 = call-dynamic "Read id.vi"("SVG Object in"=w799) -> ("id"=w798:string)  [unwired: 8 in, 2 out]
          n265 = Number To Decimal String(number=w795) -> (decimal integer string=w797:string)  [unwired: 1 in]
          n266 = Concatenate Strings("d" ("string"), w797) -> (w794:string)
        }
        n267 = Build Array (concatenate)(w778, w779, w780, w781) -> (w770:string[])
        n268 = Build Array (concatenate)(w771, w772, w773, w774) -> (w775:string[])
        n269 = Bundle By Name(cluster=w788, "Settings"=w787, "Parser"=w786, "GUIDs.Paths"=w771, "GUIDs.Rects"=w772, "GUIDs.Funnels"=w773, "GUIDs.Dots"=w774) -> (w789:T19)
        n270 = call "Populate Registry.vi"("error in"=w776, "Aliases"=w770, "Names"=w775) -> ("error out"=w777:errorcluster)  [unwired: 8 in]
        n271 = call <vilib>:"Add State(s) to Queue__jki_lib_state_machine.vi"("State(s) in (\"\")"=w793) -> ("States Out"=w792:string)  [unwired: 14 in]
      }
      frame "Integration: Change Enable" {
        # "Template Separator\n(You can make a copy of, or modify, this frame)"
        n272 = Unbundle By Name(w828) -> ("Settings"=w826:refnum<class "Setting Database.lvclass">, "Parser"=w827:refnum<class "ParseVectorFile.lvclass">)
        n273 = Unbundle By Name(w824) -> ("Items"=w823:T30[], "Enable Value"=w822:i32)
        n274 = Index Array(array=w823, index=w822) -> (element=w821:T30)
        n275 = Unbundle By Name(w821) -> ("Name"=w820:string)
        n276 = call "Setting Database.ChangeObjectEnable.vi"("error in (no error)"=w818, "ChangeObjectEnable"=w820, "Setting Database"=w826) -> ("error out"=w819:errorcluster, "Setting Database out"=w825:refnum<class "Setting Database.lvclass">)  [unwired: 7 in]
        n277 = Bundle By Name(cluster=w828, "Settings"=w825, "Parser"=w827) -> (w829:T19)
        n278 = call <vilib>:"Add State(s) to Queue__jki_lib_state_machine.vi"("State(s) in (\"\")"=w832) -> ("States Out"=w831:string)  [unwired: 14 in]
      }
      frame "Integration: Sort Paths" {
        # "Template Separator\n(You can make a copy of, or modify, this frame)"
        n279 = Unbundle By Name(w847) -> ("Settings"=w846:refnum<class "Setting Database.lvclass">, "Parser"=w845:refnum<class "ParseVectorFile.lvclass">, "Parsed Data.Paths"=w843:refnum<class "Path.lvclass">[])
        n280 = call-dynamic "Write Paths Data.vi"("error in (no error)"=w835, "Paths"=w843, "Tool Data in"=refnum<class "Tool Data.lvclass"> refnum) -> ("error out"=w839:errorcluster, "Tool Data out"=w842:refnum<class "Tool Data.lvclass">)  [unwired: 7 in]
        n281 = call "Sort Funnels and Paths.vi"("error in (no error)"=w839, "Tool Data in"=w842) -> ("error out"=w838:errorcluster, "Tool Data out"=w841:refnum<class "Tool Data.lvclass">)  [unwired: 8 in]
        n282 = call-dynamic "Read Paths Data.vi"("error in (no error)"=w838, "Tool Data in"=w841) -> ("error out"=w837:errorcluster, "Paths"=w833:refnum<class "Path.lvclass">[], "Tool Data out"=w840:refnum<class "Tool Data.lvclass">)  [unwired: 7 in]
        n283 = call-dynamic "Read Funnels Data.vi"("error in (no error)"=w837, "Tool Data in"=w840) -> ("error out"=w836:errorcluster, "Funnels"=w834:refnum<class "Path.lvclass">[])  [unwired: 7 in, 1 out]
        n284 = Bundle By Name(cluster=w847, "Settings"=w846, "Parser"=w845, "Parsed Data.Paths"=w833, "Parsed Data.Funnels"=w834) -> (w848:T19)
        n285 = call <vilib>:"Add State(s) to Queue__jki_lib_state_machine.vi"("State(s) in (\"\")"=w852) -> ("States Out"=w851:string)  [unwired: 14 in]
      }
      frame "Integration: Parser SVG" {
        # "Template Separator\n(You can make a copy of, or modify, this frame)"
        n286 = Unbundle By Name(w859) -> ("Settings"=w858:refnum<class "Setting Database.lvclass">, "Parser"=w857:refnum<class "ParseVectorFile.lvclass">)
        n287 = call "ParseVectorFile.NewFileAsynchronous.vi"("error in (no error)"=w853, "NewFile"="NewFile", "ParseVectorFile"=w857) -> ("error out"=w854:errorcluster, "ParseVectorFile out"=w856:refnum<class "ParseVectorFile.lvclass">)  [unwired: 7 in]
        n288 = Bundle By Name(cluster=w859, "Settings"=w858, "Parser"=w856) -> (w860:T19)
        n289 = call <vilib>:"Add State(s) to Queue__jki_lib_state_machine.vi"("State(s) in (\"\")"=w864) -> ("States Out"=w863:string)  [unwired: 14 in]
      }
      frame "Integration: Database Init" {
        w865 = 0
        # "Template Separator\n(You can make a copy of, or modify, this frame)"
        n290 = Unbundle By Name(w878) -> ("Settings"=w876:refnum<class "Setting Database.lvclass">, "Parser"=w880:refnum<class "ParseVectorFile.lvclass">)
        n291 = Unbundle By Name(w866) -> ("Reference"=w868:refnum<vi>)
        n292 = Unbundle By Name(w878) -> ("GUIDs.Paths"=w872:string[], "GUIDs.Rects"=w871:string[], "GUIDs.Funnels"=w869:string[], "GUIDs.Dots"=w870:string[])
        n293 = property class="MCListbox"(reference=w868, "Value"=w865) -> ()  [unwired: 1 in, 2 out]
        n294 = Bundle By Name(cluster=w866, "Value"=w865) -> (w867:refnum<class "Selector.lvclass">)
        n295 = Bundle By Name(cluster=T15 {"Paths"=[], "Rectangles"=[], "Funnels"=[], "Dots"=[]} ("Initialize"), "Paths"=w872, "Rectangles"=w871, "Funnels"=w869, "Dots"=w870) -> (w877:T15)
        n296 = call "Setting Database.Refresh.vi"("error in (no error)"=w873, "Initialize"=w877, "Setting Database"=w876) -> ("error out"=w874:errorcluster, "Setting Database out"=w875:refnum<class "Setting Database.lvclass">)  [unwired: 7 in]
        n297 = Bundle By Name(cluster=w878, "Settings"=w875, "Parser"=w880) -> (w881:T19)
        n298 = call <vilib>:"Add State(s) to Queue__jki_lib_state_machine.vi"("State(s) in (\"\")"=w884) -> ("States Out"=w883:string)  [unwired: 14 in]
      }
      frame "Integration: Stop SMOs" {
        # "Template Separator\n(You can make a copy of, or modify, this frame)"
        n299 = Unbundle By Name(w901) -> ("Settings"=w900:refnum<class "Setting Database.lvclass">, "Parser"=w899:refnum<class "ParseVectorFile.lvclass">, "Subpanel.Edit"=w890:refnum<class "Subpanel.Edit.lvclass">, "Tooler"=w885:refnum<class "Tool Data.lvclass">)
        n300 = call "Close.vi"("error in (no error)"=w888, "Subpanel.lvclass"=w890) -> ("error out"=w891:errorcluster)  [unwired: 8 in, 1 out]
        n301 = call <vilib>:"Stop.vi"("error in (no error)"=w891, "SMO"=w900) -> ("error out"=w894:errorcluster, "SMO out"=w898:refnum<class "Setting Database.lvclass">)  [unwired: 8 in]
        n302 = call <vilib>:"Stop.vi"("error in (no error)"=w888, "SMO"=w899) -> ("error out"=w893:errorcluster, "SMO out"=w897:refnum<class "ParseVectorFile.lvclass">)  [unwired: 8 in]
        n303 = call <vilib>:"Stop.vi"("error in (no error)"=w888, "SMO"=w885) -> ("error out"=w889:errorcluster, "SMO out"=w887:refnum<class "Tool Data.lvclass">)  [unwired: 8 in]
        n304 = call <vilib>:"Destroy.vi"("error in (no error)"=w894, "SMO"=w898) -> ("error out"=w896:errorcluster)  [unwired: 9 in]
        n305 = call <vilib>:"Destroy.vi"("error in (no error)"=w893, "SMO"=w897) -> ("error out"=w895:errorcluster)  [unwired: 9 in]
        n306 = call <vilib>:"Destroy.vi"("error in (no error)"=w889, "SMO"=w887) -> ("error out"=w886:errorcluster)  [unwired: 9 in]
        n307 = Merge Errors(w896, w895, w886) -> (w892:errorcluster)
        n308 = Bundle By Name(cluster=w901, "Settings"=w900, "Parser"=w899, "Tooler"=w885) -> (w902:T19)
        n309 = call <vilib>:"Add State(s) to Queue__jki_lib_state_machine.vi"("State(s) in (\"\")"=w906) -> ("States Out"=w905:string)  [unwired: 14 in]
      }
      frame "Integration: Start SMOs" {
        # "Template Separator\n(You can make a copy of, or modify, this frame)"
        n310 = Unbundle By Name(w932) -> ("Settings"=w929:refnum<class "Setting Database.lvclass">, "Parser"=w927:refnum<class "ParseVectorFile.lvclass">, "Tooler"=w911:refnum<class "Tool Data.lvclass">)
        n311 = call <vilib>:"Create.vi"("error in (no error)"=w907, "SMO"=w927) -> ("error out"=w925:errorcluster, "SMO out"=w931:refnum<class "ParseVectorFile.lvclass">)  [unwired: 7 in, 1 out]
        n312 = call <vilib>:"Create.vi"("error in (no error)"=w907, "SMO"=w911) -> ("error out"=w912:errorcluster, "SMO out"=w910:refnum<class "Tool Data.lvclass">)  [unwired: 7 in, 1 out]
        n313 = call "Setting Database Name.vi"("error in (no error)"=w907) -> ("error out"=w917:errorcluster, "Name"=w916:string)  [unwired: 9 in]
        n314 = call <vilib>:"Start.vi"("error in (no error)"=w925, "SMO"=w931) -> ("error out"=w913:errorcluster, "SMO out"=w926:refnum<class "ParseVectorFile.lvclass">)  [unwired: 8 in]
        n315 = call <vilib>:"Start.vi"("error in (no error)"=w912, "SMO"=w910) -> ("error out"=w909:errorcluster, "SMO out"=w908:refnum<class "Tool Data.lvclass">)  [unwired: 8 in]
        n316 = call <vilib>:"Create.vi"("Shared Resource (F)"=TRUE, "error in (no error)"=w917, "Subsystem Name (optional)"=w916, "SMO"=w929) -> ("error out"=w924:errorcluster, "SMO out"=w930:refnum<class "Setting Database.lvclass">)  [unwired: 5 in, 1 out]
        n317 = call <vilib>:"Start.vi"("error in (no error)"=w924, "SMO"=w930) -> ("error out"=w922:errorcluster, "SMO out"=w928:refnum<class "Setting Database.lvclass">)  [unwired: 8 in]
        n318 = control-ref of="Properties"() -> (w919:refnum<vi>)
        n319 = call "Get Manager.vi"("error in (no error)"=w922) -> ("error out"=w921:errorcluster, "Subpanel.Edit"=w920:refnum<class "Subpanel.Edit.lvclass">)  [unwired: 9 in]
        n320 = call "Initialize.vi"("error in (no error)"=w921, "Subpanel.lvclass"=w920, "Sub Panel"=w919) -> ("error out"=w914:errorcluster, "Subpanel out"=w918:refnum<class "Subpanel.Edit.lvclass">)  [unwired: 7 in]
        n321 = Merge Errors(w914, w913, w909) -> (w923:errorcluster)
        n322 = Bundle By Name(cluster=w932, "Settings"=w928, "Parser"=w926, "Subpanel.Edit"=w918, "Tooler"=w908) -> (w933:T19)
        n323 = call <vilib>:"Add State(s) to Queue__jki_lib_state_machine.vi"("State(s) in (\"\")"=w937) -> ("States Out"=w936:string)  [unwired: 14 in]
      }
      frame "---------- MCLB ----------" {
        # "Template Separator\n(You can make a copy of, or modify, this frame)"
        n324 = call <vilib>:"Add State(s) to Queue__jki_lib_state_machine.vi"("State(s) in (\"\")"=w943) -> ("States Out"=w942:string)  [unwired: 14 in]
      }
      frame "MCLB: Order Litho Data" {
        # "Template Separator\n(You can make a copy of, or modify, this frame)"
        n325 = Unbundle By Name(w946) -> ("Lithography Data"=w945:T4)
        n326 = for {
          tunnel: w945 -> [w962] mode=indexing
          tunnel: [w961] -> w954 mode=indexing
          n327 = Unbundle By Name(w962) -> ("Name"=w963:string)
          n328 = Bundle By Name(cluster=cluster{"Name":string, "Value":variant} {"Name"="", "Value"=variant} ("KVP"), "Name"=w963, "Value"=w962) -> (w961:cluster{"Name":string, "Value":variant})
        }
        n329 = call "Model--Order Key Values.vi"("error in"=w951, "KVP In"=w954, "Selector in"=w955) -> ("error out"=w950:errorcluster, "KVP Out"=w953:cluster{"Name":string, "Value":variant}[], "Selector out"=w948:refnum<class "Selector.lvclass">)  [unwired: 6 in]
        n330 = for {
          tunnel: w953 -> [w960] mode=indexing
          tunnel: [w959] -> w952 mode=indexing
          n331 = Unbundle By Name(w960) -> ("Value"=w959:variant)
        }
        n332 = Variant To Data(error in=w950, type=w945, Variant=w952) -> (data=w944:T4, error out=w949:errorcluster)
        n333 = Bundle By Name(cluster=w946, "Lithography Data"=w944) -> (w947:T19)
        n334 = call <vilib>:"Add State(s) to Queue__jki_lib_state_machine.vi"("State(s) in (\"\")"=w958) -> ("States Out"=w957:string)  [unwired: 14 in]
      }
      frame "MCLB: Generate Names" {
        # "Template Separator\n(You can make a copy of, or modify, this frame)"
        n335 = Unbundle By Name(w980) -> ("Parsed Data.Paths"=w979:refnum<class "Path.lvclass">[], "Parsed Data.Rectangles"=w976:refnum<class "Rectangle.lvclass">[], "Parsed Data.Funnels"=w974:refnum<class "Path.lvclass">[], "Parsed Data.Dots"=w972:refnum<class "Dot.lvclass">[])
        n336 = Unbundle By Name(w968) -> ("Reference"=w967:refnum<vi>)
        n337 = Array Size(array=w976) -> (size(s)=w975:i32)
        n338 = Array Size(array=w972) -> (size(s)=w971:i32)
        n339 = Array Size(array=w979) -> (size(s)=w978:i32)
        n340 = Array Size(array=w974) -> (size(s)=w973:i32)
        n341 = Build Array(w978, w975, w973, w971) -> (w977:i32[])
        n342 = for {
          tunnel: w977 -> [w987] mode=indexing
          tunnel: string[] ["p", "r", "f", "d"] -> [w986] mode=indexing
          tunnel: [w985] -> w966 mode=concatenating
          n343 = for {
            N: w987 -> [_]
            tunnel: w986 -> [w991]
            tunnel: [w989] -> w985 mode=indexing
            i -> [w993]
            n344 = Number To Decimal String(number=w993) -> (decimal integer string=w992:string)  [unwired: 1 in]
            n345 = Concatenate Strings(w991, w992) -> (w990:string)
            n346 = Bundle By Name(cluster=T9 {"Name"="", "Group"="", "Enabled"=FALSE} ("element"), "Name"=w990) -> (w989:T9)
          }
        }
        n347 = call "Items to MCLB Item Names.vi"("Items"=w966) -> ("Item Names"=w965:string[][])  [unwired: 6 in]
        n348 = Bundle By Name(cluster=w968, "Items"=w966) -> (w969:refnum<class "Selector.lvclass">)
        n349 = property class="MCListbox"(reference=w967, "ItemNames"=w965) -> ()  [unwired: 1 in, 2 out]
        n350 = call <vilib>:"Add State(s) to Queue__jki_lib_state_machine.vi"("State(s) in (\"\")"=w984) -> ("States Out"=w983:string)  [unwired: 14 in]
      }
      frame "MCLB: Reorder" {
        # "Template Separator\n(You can make a copy of, or modify, this frame)"
        n351 = Unbundle By Name(w1003) -> ("Item Names"=w1000:string[][])
        n352 = Index Array(array=w1000, index (col)=0 ("disabled index (col)")) -> (element=w998:string[])  [unwired: 1 in]
        n353 = Unbundle By Name(w996) -> ("Items"=w1002:T30[])
        n354 = call "Items to Names.vi"("Items"=w1002) -> ("Names"=w1001:string[])  [unwired: 6 in]
        n355 = for {
          tunnel: w1002 -> [w1009]
          tunnel: w1001 -> [w1011]
          tunnel: w998 -> [w1010] mode=indexing
          tunnel: [w1007] -> w995 mode=indexing
          n356 = Search 1D Array(1D array=w1011, element=w1010) -> (index of element=w1008:i32)  [unwired: 1 in]
          n357 = Index Array(array=w1009, index=w1008) -> (element=w1007:T30)
        }
        n358 = Bundle By Name(cluster=w996, "Items"=w995) -> (w997:refnum<class "Selector.lvclass">)
        n359 = call <vilib>:"Add State(s) to Queue__jki_lib_state_machine.vi"("State(s) in (\"\")"=w1006) -> ("States Out"=w1005:string)  [unwired: 14 in]
      }
      frame "MCLB: Populate New" {
        # "Template Separator\n(You can make a copy of, or modify, this frame)"
        n360 = Unbundle By Name(w1017) -> ("Item Names"=w1016:string[][])
        n361 = Index Array(array=w1016, index (col)=0 ("index (row)")) -> (element=w1014:string[])  [unwired: 1 in]
        n362 = call-dynamic "Compare New Values.vi"("error in (no error)"=w1018, "New Values"=w1014, "Selector in"=w1020) -> ("error out"=w1019:errorcluster, "Unchanged ?"=→"Unchanged?":bool, "Selector out"=w1021:refnum<class "Selector.lvclass">)  [unwired: 6 in]
        n363 = call <vilib>:"Add State(s) to Queue__jki_lib_state_machine.vi"("State(s) in (\"\")"=w1023) -> ("States Out"=w1022:string)  [unwired: 14 in]
      }
      frame "MCLB: SCM Selection" {
        # "Your code here.\n(You can make a copy of, or modify, this frame)"
        n364 = Unbundle By Name(w1024) -> ("menu path"=w1032:string)
        n365 = Unbundle By Name(w1024) -> ("Settings"=w1028:refnum<class "Setting Database.lvclass">)
        n366 = case shown="\"remove\"" w1034 {
          tunnel: w1025 -> [w1039 w1054 w1058 w1079]
          tunnel: [w1039 w1050 w1057 w1073] -> w1033
          tunnel: w1032 -> [_ w1053 _ _]
          tunnel: w1030 -> [w1038 w1052 w1055 w1078]
          tunnel: [w1038 w1044 w1061 w1074] -> w1031
          tunnel: w1028 -> [w1037 w1048 w1063 w1076]
          tunnel: [w1037 w1049 w1062 w1077] -> w1027
          frame Default {
          }
          frame "add" {
            n367 = call "Add Item to Group.vi"("error in (no error)"=w1052, "Menu Path"=w1053, "Selector in"=w1054) -> ("error out"=w1045:errorcluster, "Selector out"=w1050:refnum<class "Selector.lvclass">)  [unwired: 5 in, 2 out]
            n368 = Unbundle By Name(w1050) -> ("Items"=w1041:T30[], "Menu Index"=w1040:i32)
            n369 = Index Array(array=w1041, index=w1040) -> (element=w1051:T30)
            n370 = Unbundle By Name(w1051) -> ("Name"=w1043:string, "Group"=w1042:string)
            n371 = Bundle By Name(cluster=T16 {"Name"="", "Group"=""} ("Add To Group"), "Name"=w1043, "Group"=w1042) -> (w1046:T16)
            n372 = call "Setting Database.AddToGroup.vi"("error in (no error)"=w1045, "Add To Group"=w1046, "Setting Database"=w1048) -> ("error out"=w1044:errorcluster, "Setting Database out"=w1049:refnum<class "Setting Database.lvclass">)  [unwired: 7 in]
          }
          frame "create" {
            n373 = call-dynamic "Create New Group.vi"("error in (no error)"=w1055, "Selector in"=w1058) -> ("error out"=w1056:errorcluster, "Selector out"=w1057:refnum<class "Selector.lvclass">)  [unwired: 6 in, 2 out]
            n374 = Unbundle By Name(w1057) -> ("Items"=w1065:T30[], "Menu Index"=w1064:i32)
            n375 = Index Array(array=w1065, index=w1064) -> (element=w1068:T30)
            n376 = Unbundle By Name(w1068) -> ("Name"=w1067:string, "Group"=w1066:string)
            n377 = Bundle By Name(cluster=T17 {"Name"="", "Group"=""} ("Create New Group"), "Name"=w1067, "Group"=w1066) -> (w1060:T17)
            n378 = call "Setting Database.CreateNewGroup.vi"("error in (no error)"=w1056, "Create New Group"=w1060, "Setting Database"=w1063) -> ("error out"=w1061:errorcluster, "Setting Database out"=w1062:refnum<class "Setting Database.lvclass">)  [unwired: 7 in]
          }
          frame "remove" {
            n379 = call-dynamic "Remove Item From Group.vi"("error in (no error)"=w1078, "Selector in"=w1079) -> ("error out"=w1075:errorcluster, "Selector out"=w1073:refnum<class "Selector.lvclass">)  [unwired: 7 in, 1 out]
            n380 = Unbundle By Name(w1073) -> ("Items"=w1072:T30[], "Menu Index"=w1071:i32)
            n381 = Index Array(array=w1072, index=w1071) -> (element=w1070:T30)
            n382 = Unbundle By Name(w1070) -> ("Name"=w1069:string)
            n383 = call "Setting Database.RemoveFromGroup.vi"("error in (no error)"=w1075, "Remove From Group"=w1069, "Setting Database"=w1076) -> ("error out"=w1074:errorcluster, "Setting Database out"=w1077:refnum<class "Setting Database.lvclass">)  [unwired: 7 in]
          }
        }
        n384 = Bundle By Name(cluster=w1024, "Settings"=w1027) -> (w1026:T19)
        n385 = call <vilib>:"Add State(s) to Queue__jki_lib_state_machine.vi"("State(s) in (\"\")"=w1036) -> ("States Out"=w1035:string)  [unwired: 14 in]
      }
    }
    n386 = Empty String/Path?(string/path=w17) -> (empty?=w16:bool)
    n387 = Greater Than 0?(x=w11) -> (x > 0?=w10:bool)
    n388 = Not(x=w16) -> (.not. x?=w12:bool)
  }
  "error out" <- w4
  "Selector out" <- w6
  "Events" <- w3
  "Array" <- w2
  "Array 2" <- w1
